vi "Wide Field Drift Correction.vi"(7 "Calling VI Ref":refnum<vi>) -> ()   [LabVIEW 2016]
uses:
  Hardware Configuration/Hardware Configuration Controls/Device Type.ctl
  Hardware Configuration/Hardware Configuration Controls/Device Function.ctl
  WFDC Controls/WFDC Notifier Element.ctl
  WFDC Controls/WFDC Actions.ctl
  <vilib>/vision/Image Controls.llb/IMAQ Image.ctl
  WFDC Controls/WFDC External Sync.ctl
  WFDC Controls/WFDC Cycle Pause.ctl
  WFDC Controls/WFDC Status.ctl
  WFDC Controls/WFDC Default XY Stage Settings.ctl
  <vilib>/Utility/miscctls.llb/LVPointTypeDef.ctl
  Device Library/Cameras/IDS/IDS Controls/IDS Actions.ctl
  Device Library/Cameras/IDS/IDS Controls/IDS Parameters.ctl
  Device Library/Cameras/IDS/IDS Controls/IDS Parameter List.ctl
  Device Library/Cameras/IDS/IDS Controls/IDS ROI.ctl
  Device Library/Cameras/IDS/IDS Controls/IDS IMAQ Key Info.ctl
  Device Library/Stages/Stages Controls/Stage Actions.ctl
  Tools/TIFF Image Read and Write/ImageJ TIF Type Defs/TIF Write Image Information.ctl
  Device Library/Cameras/Camera Controls/Camera IMAQ Key Info.ctl
panel:
  in  "Main Tab":T1(tab)
  out "Remote Start":bool
  out "Running":bool
  out "Z Drift (µm)":dbl=1.0 format="%.3g"
  out "Axis 2 Drift (Pixels)":dbl=1.0 format="%.3g"
  out "Axis 1 Drift (Pixels)":dbl=1.0 format="%.3g"
  out "Z Stage Position":dbl(graph)
  out "Z Drift Amount":dbl(graph)
  out "XY Drift Correction Active":bool
  out "Error":bool
  in  "Setup New":bool
  in  "Find Focus":bool
  in  "Z Step Correction Limit (µm)":dbl=0.2
  in  "Stage Defaults":bool
  in  "Invert Y Axis":bool
  in  "Invert X Axis":bool
  in  "Flip XY Axis":bool
  in  "Frame Accumulations":u16=20
  in  "Calibration Scan Range (µm)":dbl=1.0
  in  "Log Drift Data":bool
  in  "Save Drift Images":bool
  in  "Cycle Sync XY Correction":bool
  in  "Track XY Drift":bool
  in  "Correct XY Drift":bool
  in  "XY Drift Threshold (pixels)":dbl=0.2
  in  "XY Drift Step (µm)":dbl=0.1
  in  "Z Position Offset (µm)":dbl
  in  "Z Drift Threshold (µm)":dbl=0.02
  in  "Correct Z Drift":bool=TRUE
  in  "Abort Capture If Error":bool=TRUE
  in  "Cycle Sync Z Correction":bool
  out "XY Correction Step":i32=1
  out "Correction Step":u8=1
  in  "CC Range (pixels)":i32=25 min=1 max=200
  out "CC Fit":dbl[][](graph)
  out "CC Image":dbl[][](graph)
  in  "Abort Remote":bool
  in  "CC Threshold":dbl=0.2
  in  "Fit Roundess Threshold":dbl=1.75
  out "Axis 1":dbl=1.0 format="%.3g"
  out "Axis 2":dbl=1.0 format="%.3g"
  out "Z Drift":dbl=1.0 format="%.3g"
  out "Error Message":string
  out "XY Active":bool
  out "Z Active":bool
  out "Current Frame":u32=1
  in  "Capture":bool
  in  "Number of Frames":u32=1
  in  "Image Save Path":path
  in  "Exposure Time (ms)":dbl
  in  "Image Display":bool
  in  "Live Preview":bool
  in  "Quit":bool
  # "General Settings"
  # "XY Stage Settings"
  # "XY Drift Settings"
  # "Z Drift Settings"
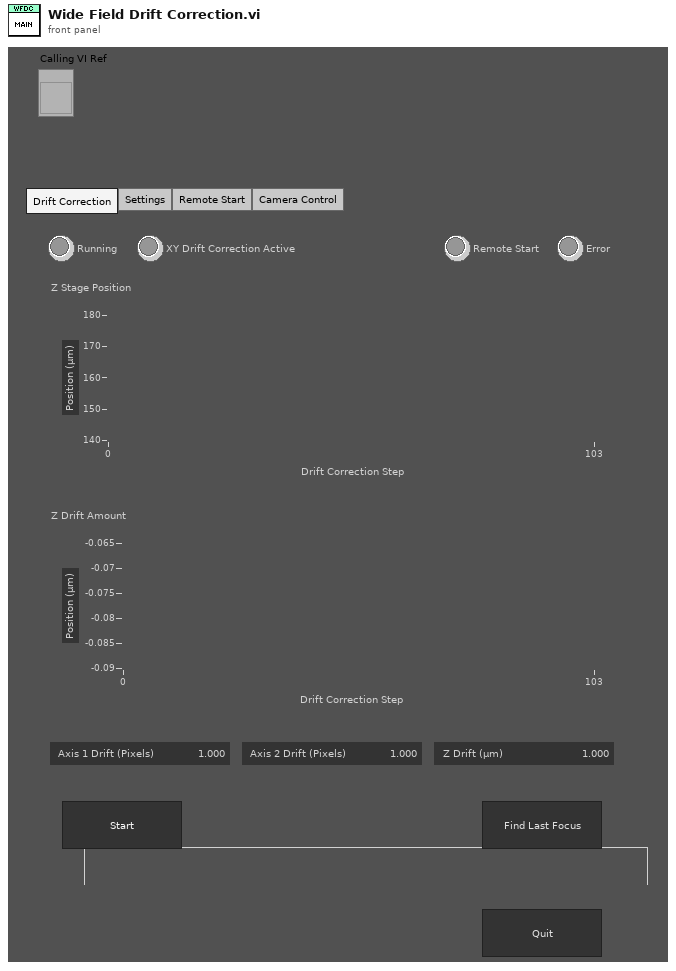
[diagram p1: front panel]
types:
  T1 = enum32{"Drift Correction", "Settings", "Remote Start", "Camera Control"}
  T2 = enum16{"Always On", "Always Off", "Off While Running"}
  T3 = typedef "LVPointTypeDef.ctl" = cluster{"Horizontal":i16, "Vertical":i16}
  T4 = typedef "IMAQ Image.ctl" = refnum<image>
  T5 = cluster{"Image Ref":T4, "Cycle Number":u16, "Camera Running?":bool, "Capture?":bool}
  T6 = typedef "WFDC Default XY Stage Settings.ctl" = cluster{"Flip XY":bool, "Invert X":bool, "Invert Y":bool}
  T7 = typedef "WFDC Cycle Pause.ctl" = enum16{"Pause Requested", "Paused", "Resume Requested", "Resumed"}
  T8 = typedef "WFDC Status.ctl" = enum16{"Idle", "Busy", "DC Active", "Error", "Canceled"}
  T9 = typedef "WFDC External Sync.ctl" = cluster{"Cycle Sync":T7, "Z Offset":dbl, "WFDC Status":T8}
  T10 = typedef "WFDC Actions.ctl" = enum16{"Error Check", "Remote Start", "Find Focus", "Pre Correct Z", "Pre Correct XY", "Setup New DC", "Setup Camera", "Get Ref Images", "Calc Calibration", "Setup Data Log", "Switch Tabs", "Get Drift / Correct Z", "Correct XY Drift", "Start Cycle", "Stop DC", "Abort Remote", "Exit Loop", "Set Error", "Generate Calibration", "Quit"}
  T11 = typedef "WFDC Notifier Element.ctl" = cluster{"WFDC Actions":T10, "Initial XYZ Positions":dbl[], "Ref Images":T4[], "Calibration (slope, inter)":dbl[], "Log Drift?":bool, "Save WF Images?":bool, "Drift Image File Ref":refnum<file>, "Drift Positions File Ref":refnum<file>, "Base Path":path, "Latest Scan Path":path, "Error":errorcluster}
  T12 = typedef "Device Function.ctl" = enum16{"Primary", "Secondary", "Overview", "Wide Field Drift Correction", "642 nm Excitation", "560 nm Excitation", "940 nm Excitation", "546 nm Excitation", "488 nm Excitation", "405 nm Excitation", "Objective Drift Correction", "4Pi Objective Lock", "Objective XY", "Objective Z", "Sample XY", "Sample Coarse Z", "Sample Z", "4Pi Lower", "4Pi Upper", "Mojo", "Adj Cavity", "Line Scanning", "Alert"}
  T13 = typedef "Device Type.ctl" = enum16{"AOTF", "Camera", "Deformable Mirror", "Laser", "Shutter", "Stage", "Waveform", "FPGA", "Email", "Filter Wheel"}
  T14 = typedef "LVRectTypeDef.ctl" = cluster{"Left":i16, "Top":i16, "Right":i16, "Bottom":i16}
  T15 = typedef "LVBoundsTypeDef.ctl" = cluster{"Width":u32, "Height":u32}
  T16 = enum8{"Enabled", "Disabled", "Disabled and Grayed Out"}
  T17 = typedef "IDS Actions.ctl" = enum16{"Error Check", "Initialize", "Preview", "Record", "Abort", "Record Settings", "Set Parameter", "Get Parameter", "Set ROI", "Get ROI", "Status", "Quit"}
  T18 = typedef "IDS Parameter List.ctl" = enum16{"Exposure Time (s)", "Binning"}
  T19 = typedef "IDS Parameters.ctl" = cluster{"Parameter":T18, "Value":dbl}
  T20 = typedef "IDS ROI.ctl" = cluster{"H Offset":i32, "V Offset":i32, "H Width":i32, "V Width":i32}
  T21 = typedef "IDS IMAQ Key Info.ctl" = cluster{"Frame":u32, "Sensor Height":i32, "Sensor Width":i32, "ROI Height":i32, "ROI Width":i32, "ROI Enable?":bool, "Bit per Pixel":u8}
  T22 = typedef "Stage Actions.ctl" = enum16{"Get Position", "MVR", "MOVE", "HALT", "ONTARGET", "ERROR", "REFERENCE", "INIT", "VELOCITY", "STATUS", "EXIT", "HOME", "ZEROPOS", "NANOPOS", "ANALOG", "QUIT"}
  T23 = enum16{"open", "replace", "create", "open or create", "replace or create", "replace or create with confirmation"}
  T24 = typedef "TIF Write Image Information.ctl" = cluster{"Image Width (Pixels)":u32, "Image Height (Pixels)":u32, "Pixel Width (µm)":dbl, "Pixel Height (µm)":dbl, "Bits Per Sample (e.g. 16)":u32, "No. of Frames":u32, "No. of Slices":u32, "Time Step (sec)":dbl, "Z Step (µm)":dbl}
  T25 = enum32{"Page Enabled", "Page Disabled", "Page Disabled & Grayed"}
  T26 = typedef "Camera IMAQ Key Info.ctl" = cluster{"Frame":u32, "Sensor Height":i32, "Sensor Width":i32, "ROI Height":i32, "ROI Width":i32, "ROI Enable?":bool, "Bit per Pixel":u8}
  T27 = enum16{"big-endian, network order", "native, host order", "little-endian"}
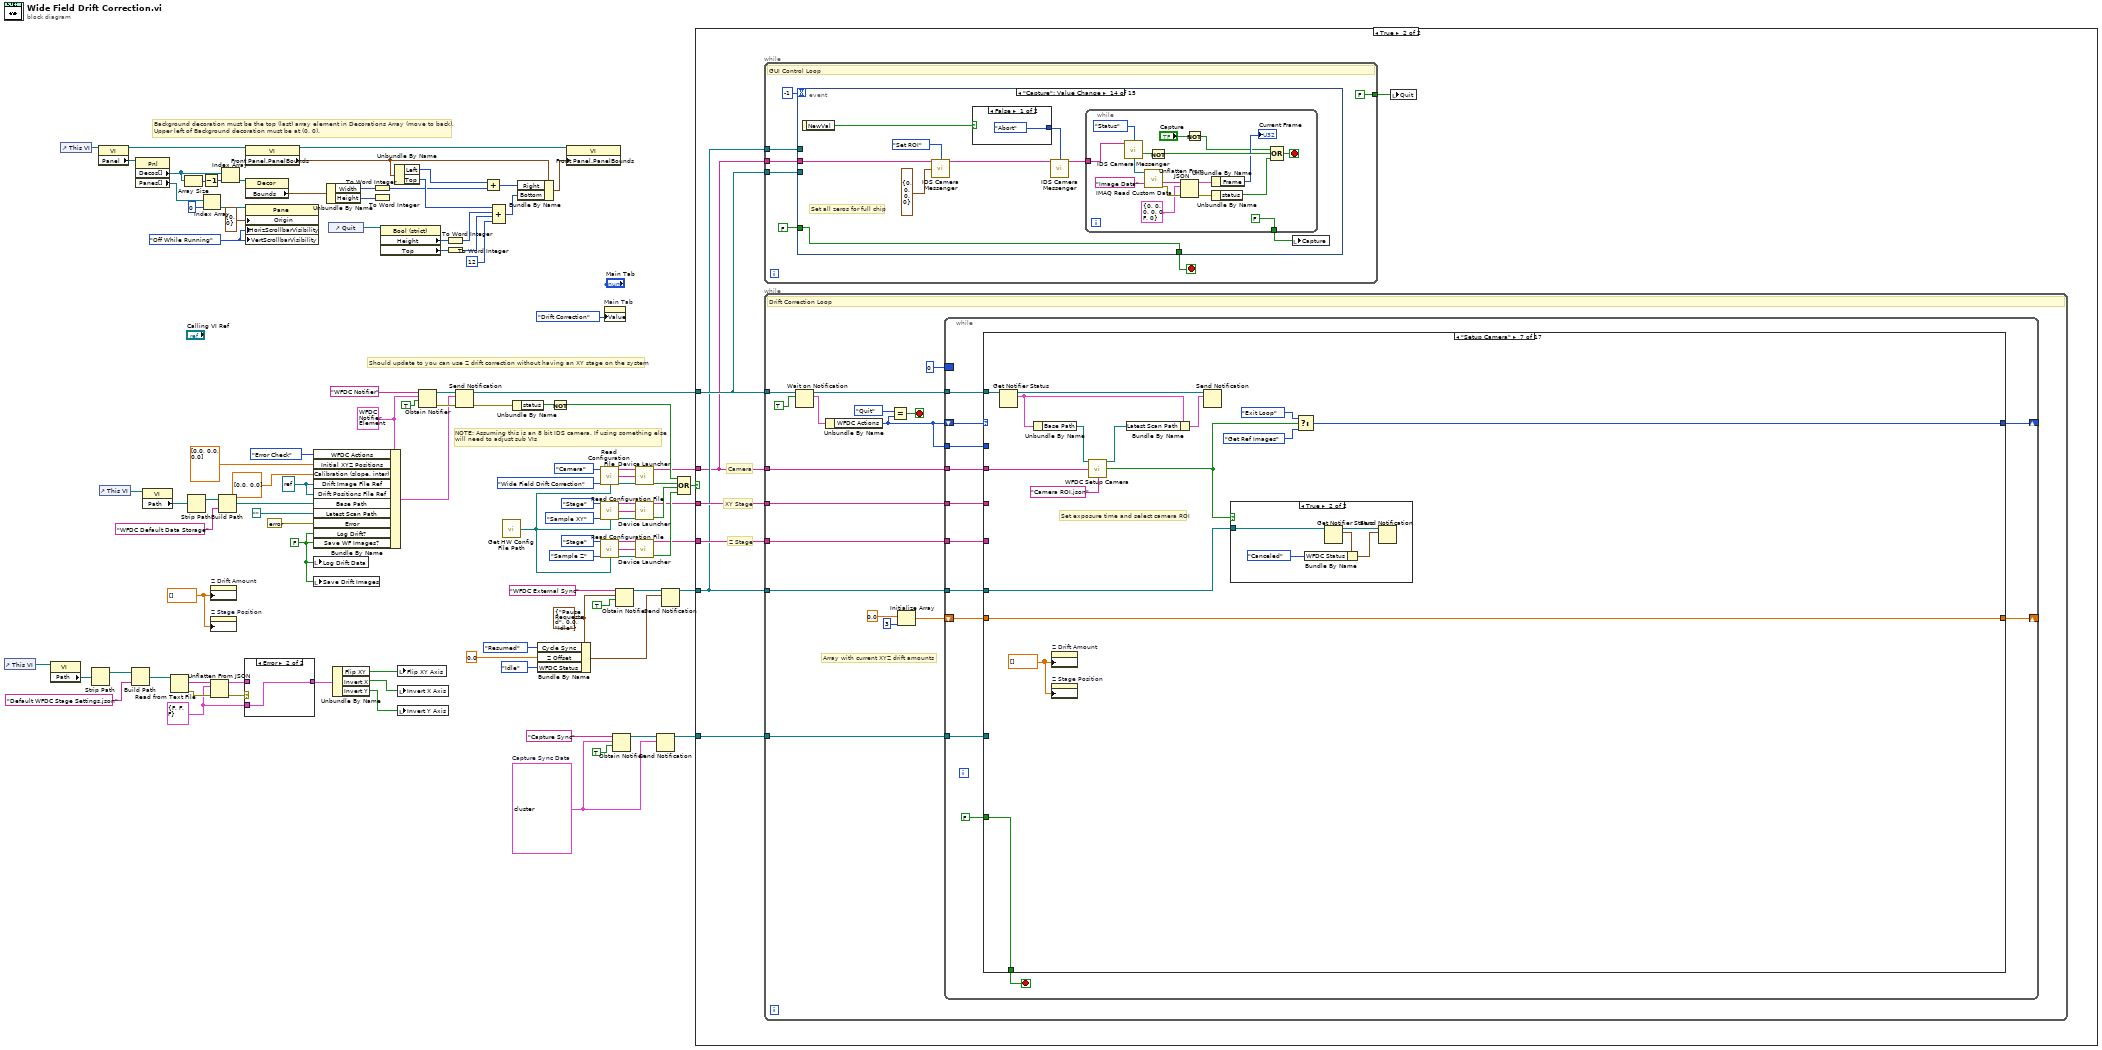
[diagram p0: block diagram]
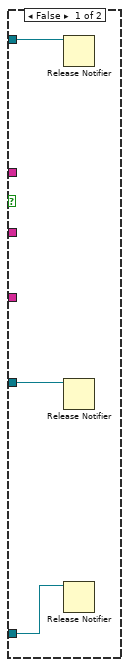
[diagram p3: hidden frame]
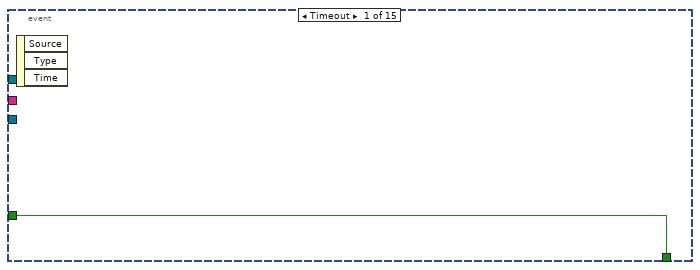
[diagram p4: hidden frame]
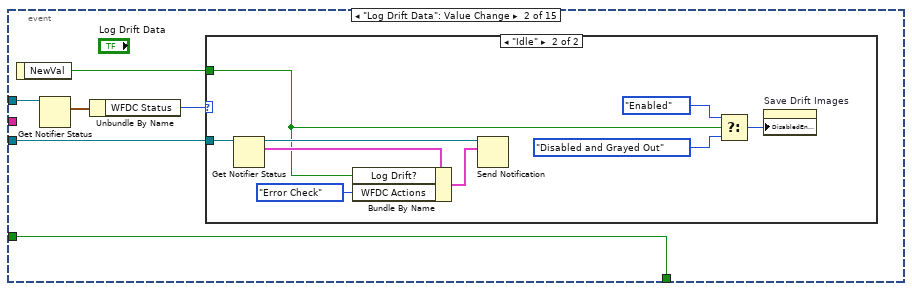
[diagram p5: hidden frame]
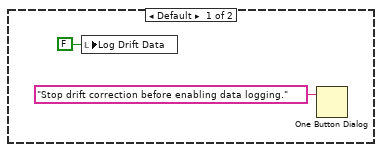
[diagram p6: hidden frame]
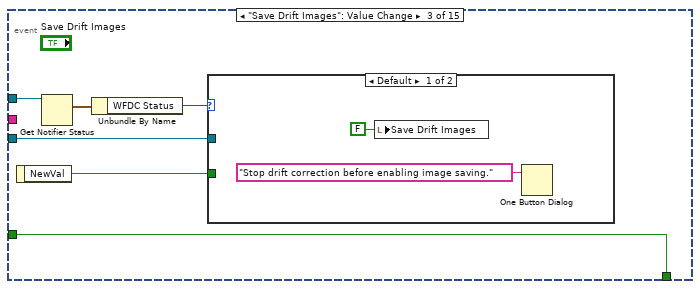
[diagram p7: hidden frame]
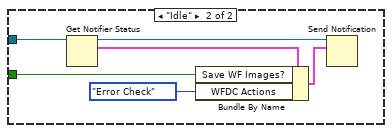
[diagram p8: hidden frame]
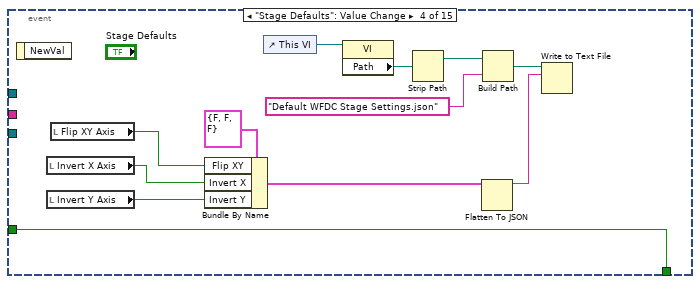
[diagram p9: hidden frame]
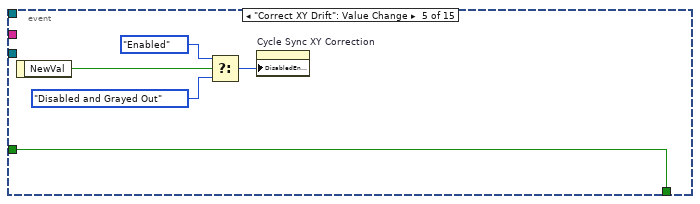
[diagram p10: hidden frame]
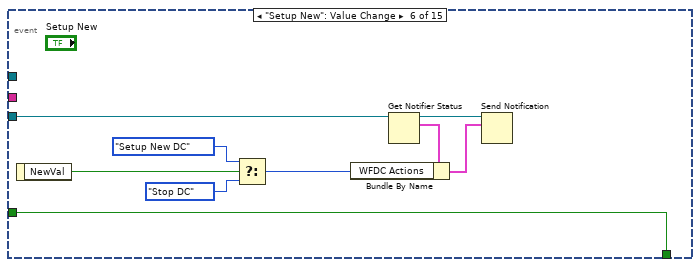
[diagram p11: hidden frame]
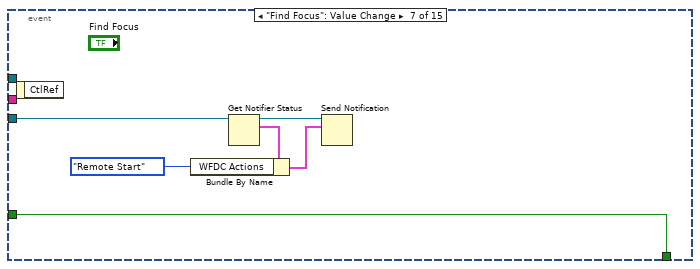
[diagram p12: hidden frame]
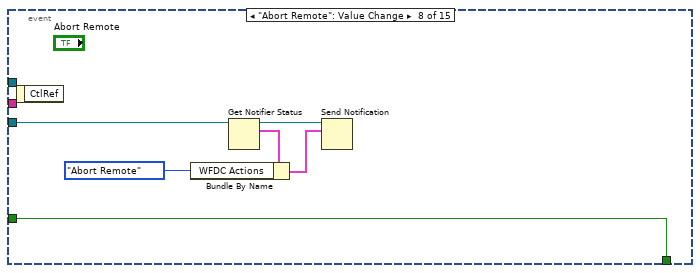
[diagram p13: hidden frame]
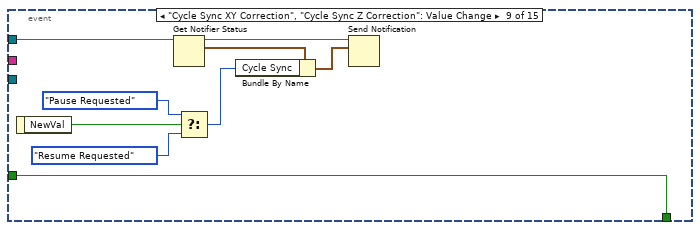
[diagram p14: hidden frame]
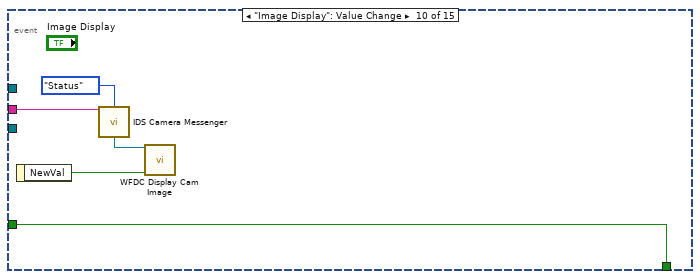
[diagram p15: hidden frame]
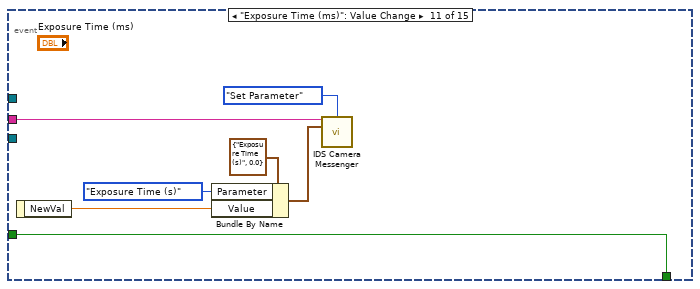
[diagram p16: hidden frame]
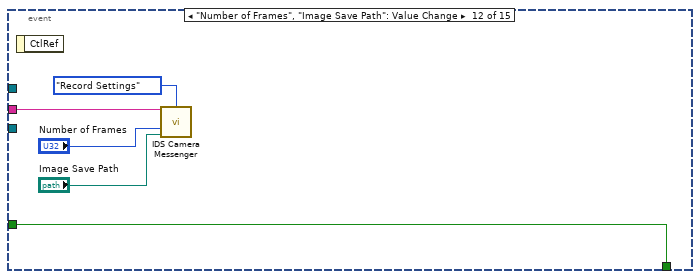
[diagram p17: hidden frame]
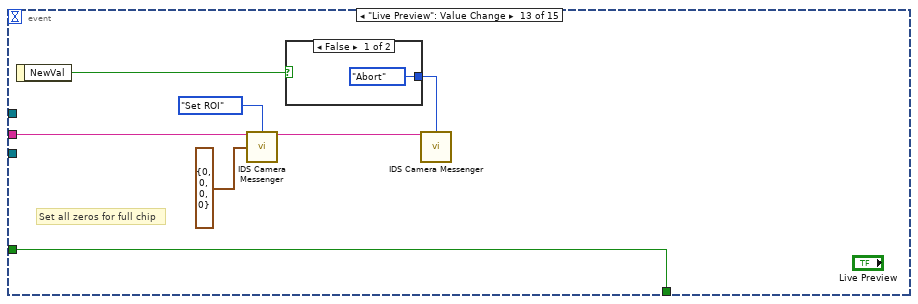
[diagram p18: hidden frame]
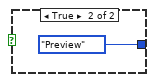
[diagram p19: hidden frame]
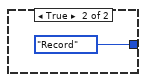
[diagram p20: hidden frame]
diagram:
  w13 = T2."Off While Running" ("Vertical Scrollbar Visibility")
  w46 = T5 {"Image Ref"=refnum, "Cycle Number"=0, "Camera Running?"=FALSE, "Capture?"=FALSE}  # Capture Sync Data
  w35 = T6 {"Flip XY"=FALSE, "Invert X"=FALSE, "Invert Y"=FALSE} ("Default WFDC Stage Settings")
  w56 = T9 {"Cycle Sync"=enum."Pause Requested", "Z Offset"=0.0, "WFDC Status"=enum."Idle"} ("WFDC External Sync")
  w64 = refnum<file> refnum ("Drift Image File Ref")
  w58 = FALSE ("Log Drift?")
  w68 = dbl[] []
  w70 = T11 {"WFDC Actions"=enum."Error Check", "Initial XYZ Positions"=[], "Ref Images"=[], "Calibration (slope, inter)"=[], "Log Drift?"=FALSE, "Save WF Images?"=FALSE, "Drift Image File Ref"=refnum, "Drift Positions File Ref"=refnum, "Base Path"=path "", "Latest Scan Path"=path "", "Error"={"status"=FALSE, "code"=0, "source"=""}} ("WFDC Notifier Element")
  # "Background decoration must be the top (last) array element in Decorations Array (move to back).\nUpper left of Background decoration must be at (0, 0)."
  # "Should update to you can use Z drift correction without having an XY stage on the system"
  # "NOTE: Assuming this is an 8 bit IDS camera. If using something else\nwill need to adjust sub VIs"
  n1 = control-ref of="This VI"() -> (w41:refnum<vi>)
  n2 = property class="VI"(reference=w41) -> ("Path"=w42:path)  [unwired: 1 in, 2 out]
  n3 = control-ref of="This VI"() -> (w5:refnum<vi>)
  n4 = Strip Path(path=w42) -> (stripped path=w43:path)  [unwired: 1 out]
  n5 = property class="VI"(reference=w5) -> (reference out=w14:refnum<vi>, "Panel"=w6:refnum<vi>)  [unwired: 1 in, 1 out]
  n6 = control-ref of="This VI"() -> (w104:refnum<vi>)
  n7 = Build Path(base path=w43, name or relative path="Default WFDC Stage Settings.json") -> (appended path=w40:path)
  n8 = property class="Pnl"(reference=w6) -> ("Decos[]"=w4:refnum<vi>[], "Panes[]"=w10:refnum<vi>[])  [unwired: 1 in, 2 out]
  n9 = property class="VI"(reference=w104) -> ("Path"=w103:path)  [unwired: 1 in, 2 out]
  n10 = Read from Text File(file (use dialog)=w40) -> (text=w39:string, error out=w38:errorcluster)  [unwired: 3 in, 2 out]
  n11 = Array Size(array=w4) -> (size(s)=w2:i32)
  n12 = Strip Path(path=w103) -> (stripped path=w102:path)  [unwired: 1 out]
  n13 = Decrement(x=w2) -> (x-1=w3:i32)
  n14 = Index Array(array=w10, index=0) -> (element=w9:refnum<vi>)
  n15 = property on="Z Drift Amount" class="WFChart (strict)"("History Data"=w68) -> ()  [unwired: 2 in, 2 out]
  n16 = property on="Z Stage Position" class="WFChart (strict)"("History Data"=w68) -> ()  [unwired: 2 in, 2 out]
  n17 = Unflatten From JSON(JSON string=w39, type and defaults=w35, error in (no error)=w38) -> (value=w36:T6, error out=w37:errorcluster)  [unwired: 4 in]
  n18 = Build Path(base path=w102, name or relative path="WFDC Default Data Storage") -> (appended path=w61:path)
  n19 = Index Array(array=w4, index=w3) -> (element=w12:refnum<vi>)
  n20 = case shown="Error" w37 {
    tunnel: w36 -> [w105 _]
    tunnel: [w105 w106] -> w34
    tunnel: w35 -> [_ w106]
    frame No Error {
    }
    frame Error {
    }
  }
  n21 = property class="VI"(reference=w14) -> (reference out=w16:refnum<vi>, "Front Panel.PanelBounds"=w17:T14)  [unwired: 1 in, 1 out]
  n22 = property class="Decor"(reference=w12) -> ("Bounds"=w15:T15)  [unwired: 1 in, 2 out]
  n23 = property class="Pane"(reference=w9, "Origin"=T3 {"Horizontal"=0, "Vertical"=0}, "HorizScrollbarVisibility"=w13, "VertScrollbarVisibility"=w13) -> ()  [unwired: 1 in, 2 out]
  n24 = Bundle By Name(cluster=w70, "WFDC Actions"=WFDC_Actions."Error Check", "Initial XYZ Positions"=dbl[] [0.0, 0.0, 0.0], "Calibration (slope, inter)"=dbl[] [0.0, 0.0], "Drift Image File Ref"=w64, "Drift Positions File Ref"=w64, "Base Path"=w61, "Latest Scan Path"=path "", "Error"=errorcluster {"status"=FALSE, "code"=0, "source"=""}, "Log Drift?"=w58, "Save WF Images?"=w58) -> (w69:T11)
  n25 = local write "Log Drift Data"(w58) -> ()
  n26 = local write "Save Drift Images"(w58) -> ()
  n27 = Unbundle By Name(w15) -> ("Width"=w20:u32, "Height"=w23:u32)
  n28 = control-ref of="Quit"() -> (w7:refnum<vi>)
  n29 = Unbundle By Name(w34) -> ("Flip XY"=w33:bool, "Invert X"=w32:bool, "Invert Y"=w31:bool)
  n30 = To Word Integer(number=w20) -> (16bit integer=w22:i16)
  n31 = To Word Integer(number=w23) -> ()  [unwired: 1 out]
  n32 = property class="Bool (strict)"(reference=w7) -> ("Height"=w25:u32, "Top"=w26:i32)  [unwired: 1 in, 2 out]
  n33 = Unbundle By Name(w17) -> ("Left"=w19:i16, "Top"=w30:i16)
  n34 = local write "Flip XY Axis"(w33) -> ()
  n35 = local write "Invert X Axis"(w32) -> ()
  n36 = local write "Invert Y Axis"(w31) -> ()
  n37 = Obtain Notifier(name (unnamed)="WFDC Notifier", notification data type=w70, create if not found? (T)=TRUE) -> (notifier out=w84:refnum<notifier>, error out=w82:errorcluster)  [unwired: 1 in, 1 out]
  n38 = To Word Integer(number=w25) -> (16bit integer=w28:i16)
  n39 = To Word Integer(number=w26) -> (16bit integer=w29:i16)
  n40 = Send Notification(notification=w69, notifier=w84, error in (no error)=w82) -> (notifier out=w83:refnum<notifier>, error out=w77:errorcluster)
  n41 = Add(x=w19, y=w22) -> (x+y=w21:i16)
  n42 = Compound Arithmetic op=ADD(w30, w28, w29, i16 12 ("y")) -> (w24:i16)
  n43 = call "Get HW Config File Path.vi"() -> ("File Path"=w66:path)  [unwired: 14 in, 1 out]
  n44 = Unbundle By Name(w77) -> ("status"=w76:bool)
  n45 = Bundle By Name(cluster=w17, "Right"=w21, "Bottom"=w24) -> (w18:T14)
  n46 = Bundle By Name(cluster=w56, "Cycle Sync"=WFDC_Cycle_Pause."Resumed", "Z Offset"=0.0, "WFDC Status"=WFDC_Status."Idle") -> (w50:T9)
  n47 = Not(x=w76) -> (.not. x?=w75:bool)
  n48 = property class="VI"(reference=w16, "Front Panel.PanelBounds"=w18) -> ()  [unwired: 1 in, 2 out]
  n49 = call "Read Configuration File.vi"("Device Type"=Device_Type."Camera", "Device Function"=Device_Function."Wide Field Drift Correction", "Config File Path"=w66) -> ("Unique Notifier Name"=w100:string, "Device Ports/IDs/Channels"=w99:string[], "Device Engine Path"=w98:path)  [unwired: 9 in, 1 out]
  n50 = call "Read Configuration File.vi"("Device Type"=Device_Type."Stage", "Device Function"=Device_Function."Sample XY", "Config File Path"=w66) -> ("Unique Notifier Name"=w91:string, "Device Ports/IDs/Channels"=w92:string[], "Device Engine Path"=w93:path)  [unwired: 9 in, 1 out]
  n51 = call "Read Configuration File.vi"("Device Type"=Device_Type."Stage", "Device Function"=Device_Function."Sample Z", "Config File Path"=w66) -> ("Unique Notifier Name"=w90:string, "Device Ports/IDs/Channels"=w89:string[], "Device Engine Path"=w88:path)  [unwired: 9 in, 1 out]
  n52 = property on="Main Tab" class="TabCtl (strict)"("Value"=T1."Drift Correction" ("Main Tab")) -> ()  [unwired: 2 in, 2 out]
  n53 = Obtain Notifier(name (unnamed)="Capture Sync", notification data type=w46, create if not found? (T)=TRUE) -> (notifier out=w47:refnum<notifier>)  [unwired: 1 in, 2 out]
  n54 = Obtain Notifier(name (unnamed)="WFDC External Sync", notification data type=w56, create if not found? (T)=TRUE) -> (notifier out=w52:refnum<notifier>)  [unwired: 1 in, 2 out]
  n55 = call "Device Launcher.vi"("Notifier Name"=w100, "Device Ports/IDs/Channels"=w99, "Device Engine Path"=w98) -> ("Notifier Name"=w73:string, "Running?"=w80:bool)  [unwired: 11 in]
  n56 = call "Device Launcher.vi"("Notifier Name"=w91, "Device Ports/IDs/Channels"=w92, "Device Engine Path"=w93) -> ("Notifier Name"=w72:string, "Running?"=w79:bool)  [unwired: 11 in]
  n57 = call "Device Launcher.vi"("Notifier Name"=w90, "Device Ports/IDs/Channels"=w89, "Device Engine Path"=w88) -> ("Notifier Name"=w71:string, "Running?"=w78:bool)  [unwired: 11 in]
  n58 = Send Notification(notification=w46, notifier=w47) -> (notifier out=w45:refnum<notifier>)  [unwired: 1 in, 1 out]
  n59 = Send Notification(notification=w50, notifier=w52) -> (notifier out=w51:refnum<notifier>)  [unwired: 1 in, 1 out]
  n60 = Compound Arithmetic op=OR(w75, w80, w79, w78) -> (w74:bool)
  n61 = case shown="True" w74 {
    tunnel: w83 -> [w109 w114]
    tunnel: w73 -> [_ w110]
    tunnel: w72 -> [_ w116]
    tunnel: w71 -> [_ w115]
    tunnel: w51 -> [w108 w112]
    tunnel: w45 -> [w107 w111]
    frame False {
      n62 = Release Notifier(notifier=w109) -> ()  [unwired: 2 in, 3 out]
      n63 = Release Notifier(notifier=w108) -> ()  [unwired: 2 in, 3 out]
      n64 = Release Notifier(notifier=w107) -> ()  [unwired: 2 in, 3 out]
    }
    frame True {
      # "Z Stage"
      # "XY Stage"
      # "Camera"
      n65 = while {
        tunnel: w114 -> [w120]
        tunnel: [FALSE] -> w113
        tunnel: w112 -> [w118]
        tunnel: w110 -> [w117]
        stop <- w123 stop-if-true
        # "GUI Control Loop"
        n66 = event shown="[13] \"Capture\": Value Change" {
          selector: _ -> [_ _ _ _ _ _ _ _ _ _ _ _ _ _ _]
          dyn-events: _ -> [_ _ _ _ _ _ _ _ _ _ _ _ _ _ _]
          timeout: -1 -> [_ _ _ _ _ _ _ _ _ _ _ _ _ _ _]
          tunnel: [w124 w130 w147 w167 w168 w181 w187 w193 w202 w205 w214 w219 w226 w230 w258] -> w123
          tunnel: FALSE -> [w124 w130 w147 w167 w168 w181 w187 w193 w202 w205 w214 w219 w226 w230 _]
          tunnel: w120 -> [_ w129 w146 _ _ w177 w182 w188 _ _ _ _ _ _ w264]
          tunnel: w118 -> [_ w127 w143 _ _ _ _ _ w200 _ _ _ _ _ w262]
          tunnel: w117 -> [_ _ _ _ _ _ _ _ _ w206 w209 w215 w221 w235 _]
          event Timeout {
            n67 = event-data() -> ()  [unwired: 1 in, 3 out]
          }
          event "Log Drift Data": Value Change {
            n68 = event-data() -> ("NewVal"=w128:bool)  [unwired: 1 in]
            n69 = Get Notifier Status(notifier=w127) -> (current notification=w126:T9)  [unwired: 1 in, 4 out]
            n70 = Unbundle By Name(w126) -> ("WFDC Status"=w125:T8)
            n71 = case shown="\"Idle\"" w125 {
              tunnel: w129 -> [_ w140]
              tunnel: w128 -> [_ w133]
              frame Default {
                n72 = local write "Log Drift Data"(FALSE ("Log Drift Data")) -> ()
                n73 = One Button Dialog(message="Stop drift correction before enabling data logging.") -> ()  [unwired: 1 in, 1 out]
              }
              frame "Idle" {
                n74 = Get Notifier Status(notifier=w140) -> (notifier out=w141:refnum<notifier>, current notification=w139:T11)  [unwired: 1 in, 3 out]
                n75 = Bundle By Name(cluster=w139, "Log Drift?"=w133, "WFDC Actions"=WFDC_Actions."Error Check") -> (w137:T11)
                n76 = Send Notification(notification=w137, notifier=w141) -> ()  [unwired: 1 in, 2 out]
                n77 = Select(t=T16."Enabled" ("Disabled"), s=w133, f=T16."Disabled and Grayed Out" ("Disabled")) -> (s? t:f=w134:T16)
                n78 = property on="Save Drift Images" class="Bool (strict)"("DisabledEnum"=w134) -> ()  [unwired: 2 in, 2 out]
              }
            }
          }
          event "Save Drift Images": Value Change {
            n79 = event-data() -> ("NewVal"=w145:bool)  [unwired: 1 in]
            n80 = Get Notifier Status(notifier=w143) -> (current notification=w144:T9)  [unwired: 1 in, 4 out]
            n81 = Unbundle By Name(w144) -> ("WFDC Status"=w142:T8)
            n82 = case shown="Default" w142 {
              tunnel: w146 -> [_ w154]
              tunnel: w145 -> [_ w152]
              frame Default {
                n83 = local write "Save Drift Images"(FALSE ("Save Drift Images")) -> ()
                n84 = One Button Dialog(message="Stop drift correction before enabling image saving.") -> ()  [unwired: 1 in, 1 out]
              }
              frame "Idle" {
                n85 = Get Notifier Status(notifier=w154) -> (notifier out=w155:refnum<notifier>, current notification=w153:T11)  [unwired: 1 in, 3 out]
                n86 = Bundle By Name(cluster=w153, "Save WF Images?"=w152, "WFDC Actions"=WFDC_Actions."Error Check") -> (w150:T11)
                n87 = Send Notification(notification=w150, notifier=w155) -> ()  [unwired: 1 in, 2 out]
              }
            }
          }
          event "Stage Defaults": Value Change {
            n88 = event-data() -> ()  [unwired: 1 in, 1 out]
            n89 = local read "Invert X Axis"() -> (w157:bool)
            n90 = local read "Invert Y Axis"() -> (w158:bool)
            n91 = local read "Flip XY Axis"() -> (w156:bool)
            n92 = Bundle By Name(cluster=T6 {"Flip XY"=FALSE, "Invert X"=FALSE, "Invert Y"=FALSE} ("Default WFDC Stage Settings"), "Flip XY"=w156, "Invert X"=w157, "Invert Y"=w158) -> (w159:T6)
            n93 = control-ref of="This VI"() -> (w166:refnum<vi>)
            n94 = property class="VI"(reference=w166) -> ("Path"=w165:path)  [unwired: 1 in, 2 out]
            n95 = Strip Path(path=w165) -> (stripped path=w164:path)  [unwired: 1 out]
            n96 = Flatten To JSON(anything=w159) -> (JSON string=w161:string)  [unwired: 2 in, 1 out]
            n97 = Build Path(base path=w164, name or relative path="Default WFDC Stage Settings.json") -> (appended path=w162:path)
            n98 = Write to Text File(file (use dialog)=w162, text=w161) -> ()  [unwired: 2 in, 3 out]
          }
          event "Correct XY Drift": Value Change {
            n99 = event-data() -> ("NewVal"=w172:bool)  [unwired: 1 in]
            n100 = Select(t=T16."Enabled" ("Disabled"), s=w172, f=T16."Disabled and Grayed Out") -> (s? t:f=w170:T16)
            n101 = property on="Cycle Sync XY Correction" class="Bool (strict)"("DisabledEnum"=w170) -> ()  [unwired: 2 in, 2 out]
          }
          event "Setup New": Value Change {
            n102 = event-data() -> ("NewVal"=w176:bool)  [unwired: 1 in]
            n103 = Select(t=WFDC_Actions."Setup New DC" ("WFDC Actions"), s=w176, f=WFDC_Actions."Stop DC" ("WFDC Actions")) -> (s? t:f=w174:T10)
            n104 = Get Notifier Status(notifier=w177) -> (notifier out=w179:refnum<notifier>, current notification=w180:T11)  [unwired: 1 in, 3 out]
            n105 = Bundle By Name(cluster=w180, "WFDC Actions"=w174) -> (w178:T11)
            n106 = Send Notification(notification=w178, notifier=w179) -> ()  [unwired: 1 in, 2 out]
          }
          event "Find Focus": Value Change {
            n107 = event-data() -> ()  [unwired: 1 in, 1 out]
            n108 = Get Notifier Status(notifier=w182) -> (notifier out=w185:refnum<notifier>, current notification=w186:T11)  [unwired: 1 in, 3 out]
            n109 = Bundle By Name(cluster=w186, "WFDC Actions"=WFDC_Actions."Remote Start") -> (w184:T11)
            n110 = Send Notification(notification=w184, notifier=w185) -> ()  [unwired: 1 in, 2 out]
          }
          event "Abort Remote": Value Change {
            n111 = event-data() -> ()  [unwired: 1 in, 1 out]
            n112 = Get Notifier Status(notifier=w188) -> (notifier out=w191:refnum<notifier>, current notification=w192:T11)  [unwired: 1 in, 3 out]
            n113 = Bundle By Name(cluster=w192, "WFDC Actions"=WFDC_Actions."Abort Remote") -> (w190:T11)
            n114 = Send Notification(notification=w190, notifier=w191) -> ()  [unwired: 1 in, 2 out]
          }
          event "Cycle Sync XY Correction", "Cycle Sync Z Correction": Value Change {
            n115 = event-data() -> ("NewVal"=w201:bool)  [unwired: 1 in]
            n116 = Get Notifier Status(notifier=w200) -> (notifier out=w195:refnum<notifier>, current notification=w199:T9)  [unwired: 1 in, 3 out]
            n117 = Select(t=WFDC_Cycle_Pause."Pause Requested" ("Cycle Sync"), s=w201, f=WFDC_Cycle_Pause."Resume Requested" ("Cycle Sync")) -> (s? t:f=w196:T7)
            n118 = Bundle By Name(cluster=w199, "Cycle Sync"=w196) -> (w194:T9)
            n119 = Send Notification(notification=w194, notifier=w195) -> ()  [unwired: 1 in, 2 out]
          }
          event "Image Display": Value Change {
            n120 = event-data() -> ("NewVal"=w203:bool)  [unwired: 1 in]
            n121 = call "IDS Camera Messenger.vi"("Notifier Name"=w206, "IDS Actions"=IDS_Actions."Status") -> ("Image Ref"=w204:T4)  [unwired: 8 in, 5 out]
            n122 = call "WFDC Display Cam Image.vi"("Image Ref"=w204, "Display?"=w203) -> ()  [unwired: 14 in]
          }
          event "Exposure Time (ms)": Value Change {
            n123 = event-data() -> ("NewVal"=w210:dbl)  [unwired: 1 in]
            n124 = Bundle By Name(cluster=T19 {"Parameter"=enum."Exposure Time (s)", "Value"=0.0} ("IDS Parameter"), "Parameter"=IDS_Parameter_List."Exposure Time (s)", "Value"=w210) -> (w208:T19)
            n125 = call "IDS Camera Messenger.vi"("Notifier Name"=w209, "IDS Actions"=IDS_Actions."Set Parameter", "IDS Parameter"=w208) -> ()  [unwired: 7 in, 6 out]
          }
          event "Number of Frames", "Image Save Path": Value Change {
            n126 = event-data() -> ()  [unwired: 1 in, 1 out]
            n127 = call "IDS Camera Messenger.vi"("Notifier Name"=w215, "IDS Actions"=IDS_Actions."Record Settings", "# of Frames"="Number of Frames", "File Save Path"="Image Save Path") -> ()  [unwired: 6 in, 6 out]
          }
          event "Live Preview": Value Change {
            # "Set all zeros for full chip"
            n128 = event-data() -> ("NewVal"=w225:bool)  [unwired: 1 in]
            n129 = call "IDS Camera Messenger.vi"("Notifier Name"=w221, "IDS Actions"=IDS_Actions."Set ROI", "ROI Setup"=T20 {"H Offset"=0, "V Offset"=0, "H Width"=0, "V Width"=0}) -> ("Notifier Name (Dup)"=w220:string)  [unwired: 7 in, 5 out]
            n130 = case shown="False" w225 {
              tunnel: [IDS_Actions."Abort" ("IDS Actions") IDS_Actions."Preview" ("IDS Actions")] -> w224
              frame False {
              }
              frame True {
              }
            }
            n131 = call "IDS Camera Messenger.vi"("Notifier Name"=w220, "IDS Actions"=w224) -> ()  [unwired: 8 in, 6 out]
          }
          event "Capture": Value Change {
            # "Set all zeros for full chip"
            n132 = event-data() -> ("NewVal"=w237:bool)  [unwired: 1 in]
            n133 = call "IDS Camera Messenger.vi"("Notifier Name"=w235, "IDS Actions"=IDS_Actions."Set ROI", "ROI Setup"=T20 {"H Offset"=0, "V Offset"=0, "H Width"=0, "V Width"=0}) -> ("Notifier Name (Dup)"=w234:string)  [unwired: 7 in, 5 out]
            n134 = case shown="False" w237 {
              tunnel: [IDS_Actions."Abort" ("IDS Actions") IDS_Actions."Record" ("IDS Actions")] -> w236
              frame False {
              }
              frame True {
              }
            }
            n135 = call "IDS Camera Messenger.vi"("Notifier Name"=w234, "IDS Actions"=w236) -> ("Notifier Name (Dup)"=w231:string)  [unwired: 8 in, 5 out]
            n136 = while {
              tunnel: w231 -> [w254]
              tunnel: [FALSE] -> w229
              stop <- w240 stop-if-true
              n137 = call "IDS Camera Messenger.vi"("Notifier Name"=w254, "IDS Actions"=IDS_Actions."Status") -> ("Running?"=w252:bool, "Image Ref"=w246:T4)  [unwired: 8 in, 4 out]
              n138 = call "IMAQ Read Custom Data"("Key"="Image Data", "Image"=w246) -> ("error out"=w251:errorcluster, "Custom Data Out"=w248:string)  [unwired: 7 in, 1 out]
              n139 = Not(x=w252) -> (.not. x?=w244:bool)
              n140 = Unflatten From JSON(JSON string=w248, type and defaults=T21 {"Frame"=0, "Sensor Height"=0, "Sensor Width"=0, "ROI Height"=0, "ROI Width"=0, "ROI Enable?"=FALSE, "Bit per Pixel"=0} ("IDS IMAQ Key Info"), error in (no error)=w251) -> (value=w250:T21, error out=w245:errorcluster)  [unwired: 4 in]
              n141 = Not(x="Capture") -> (.not. x?=w238:bool)
              n142 = Unbundle By Name(w250) -> ("Frame"=→"Current Frame":u32)
              n143 = Unbundle By Name(w245) -> ("status"=w243:bool)
              n144 = Compound Arithmetic op=OR(w238, w244, w243) -> (w240:bool)
            }
            n145 = local write "Capture"(w229) -> ()
          }
          event "Quit": Value Change {
            n146 = event-data() -> ()  [unwired: 1 in, 1 out]
            n147 = Get Notifier Status(notifier=w264) -> (notifier out=w263:refnum<notifier>, current notification=w266:T11)  [unwired: 1 in, 3 out]
            n148 = Bundle By Name(cluster=w266, "WFDC Actions"=WFDC_Actions."Stop DC", "Log Drift?"=FALSE) -> (w265:T11)
            n149 = Send Notification(notification=w265, notifier=w263) -> (notifier out=w261:refnum<notifier>)  [unwired: 1 in, 1 out]
            n150 = while {
              tunnel: w262 -> [w288]
              tunnel: w261 -> [w287]
              tunnel: [w287] -> w260
              tunnel: [w278] -> w259
              i -> [w281]
              stop <- w279 stop-if-true
              n151 = Get Notifier Status(notifier=w288) -> (current notification=w286:T9)  [unwired: 1 in, 4 out]
              n152 = Wait (ms)(milliseconds to wait=u32 1) -> ()  [unwired: 1 out]
              n153 = Greater?(x=w281, y=10000) -> (0:w278:bool)
              n154 = Unbundle By Name(w286) -> ("WFDC Status"=w285:T8)
              n155 = Equal?(x=WFDC_Status."Idle", y=w285) -> (x = y?=w282:bool)
              n156 = Or(x=w282, y=w278) -> (x .or. y?=w279:bool)
            }
            n157 = case shown="False" w259 {
              tunnel: w260 -> [w270 _]
              tunnel: [TRUE FALSE] -> w258
              frame False {
                n158 = flat-sequence {
                  tunnel: [w276] -> w271
                  tunnel: w270 -> [w276]
                  frame #0 {
                    n159 = Wait (ms)(milliseconds to wait=u32 20) -> ()  [unwired: 1 out]
                  }
                }
                n160 = Get Notifier Status(notifier=w271) -> (notifier out=w272:refnum<notifier>, current notification=w274:T11)  [unwired: 1 in, 3 out]
                n161 = Bundle By Name(cluster=w274, "WFDC Actions"=WFDC_Actions."Quit") -> (w269:T11)
                n162 = Send Notification(notification=w269, notifier=w272) -> ()  [unwired: 1 in, 2 out]
              }
              frame True {
              }
            }
          }
        }
      }
      n163 = while {
        tunnel: w114 -> [w304]
        tunnel: w110 -> [w296]
        tunnel: w116 -> [w299]
        tunnel: w115 -> [w298]
        tunnel: w112 -> [w291]
        tunnel: w111 -> [w290]
        stop <- w300 stop-if-true
        # "Array with current XYZ drift amounts"
        # "Drift Correction Loop"
        n164 = Wait on Notification(notifier=w304, ignore previous (F)=TRUE) -> (notifier out=w303:refnum<notifier>, notification=w302:T11)  [unwired: 2 in, 2 out]
        n165 = Unbundle By Name(w302) -> ("WFDC Actions"=w297:T10)
        n166 = Equal?(x=WFDC_Actions."Quit", y=w297) -> (x = y?=w300:bool)
        n167 = Initialize Array(0.0 ("element"), 3 ("dimension size")) -> (w294:dbl[])
        n168 = while {
          tunnel: w303 -> [w309]
          shift-right: [w313] -> _
          shift-left: w297 -> [w317]
          tunnel: w296 -> [w316]
          tunnel: w299 -> [w315]
          tunnel: w298 -> [w314]
          tunnel: w297 -> [w310]
          tunnel: w291 -> [w308]
          shift-right: [w306] -> _
          shift-left: w294 -> [w307]
          tunnel: w290 -> [w305]
          border: u8 0 -> [_]
          stop <- w311 stop-if-true
          n169 = case shown="\"Setup Camera\"" w317 {
            selector: w317 -> [_ _ _ _ _ _ _ _ _ _ _ _ _ _ w1062 _ _]
            tunnel: w316 -> [_ w356 w409 w472 w534 _ w683 w726 w762 w816 _ w912 _ _ w1077 _ _]
            tunnel: w315 -> [_ _ w396 w469 w541 _ _ w719 _ _ _ _ w971 _ _ _ _]
            tunnel: w314 -> [_ _ w408 w468 _ _ _ w716 _ _ _ w897 _ _ _ _ _]
            tunnel: [WFDC_Actions."Exit Loop" ("x") w350 w379 w461 w519 w663 w691 WFDC_Actions."Calc Calibration" ("x") w733 WFDC_Actions."Switch Tabs" ("x") WFDC_Actions."Get Drift / Correct Z" ("x") w855 w961 WFDC_Actions."Get Drift / Correct Z" ("x") WFDC_Actions."Exit Loop" ("x") WFDC_Actions."Exit Loop" ("x") WFDC_Actions."Quit" ("x")] -> w313
            tunnel: FALSE -> [w320 w372 w411 w476 w546 w664 w693 w727 w766 w817 w824 w916 w972 w1026 w1078 _ _]
            tunnel: [w320 w372 w411 w476 w546 w664 w693 w727 w766 w817 w824 w916 w972 w1026 w1078 TRUE TRUE] -> w311
            tunnel: w310 -> [_ _ _ _ _ w656 _ _ w737 _ _ _ _ _ _ _ _]
            tunnel: w309 -> [_ w371 w404 w475 w543 _ w687 w725 w765 w818 _ w915 _ _ w1074 _ w1094]
            tunnel: w308 -> [_ w341 w381 _ w536 w658 w679 _ w750 _ _ w886 w963 w1024 w1064 _ w1093]
            tunnel: w307 -> [w318 w342 w405 w470 w542 w662 w689 w706 w760 w809 w831 w908 w964 w1027 w1069 w1086 w1092]
            tunnel: [w318 w342 w405 w470 w542 w662 w689 w706 w760 w809 w831 w892 w964 w1027 w1069 w1086 w1092] -> w306
            tunnel: w305 -> [_ _ _ _ _ _ _ _ _ _ _ w883 _ w1023 _ _ w1089]
            frame "Error Check", Default {
            }
            frame "Remote Start" {
              n170 = Get Notifier Status(notifier=w371) -> (notifier out=w363:refnum<notifier>, current notification=w366:T11, error out=w351:errorcluster)  [unwired: 1 in, 2 out]
              n171 = Unbundle By Name(w366) -> ("Latest Scan Path"=w343:path)
              n172 = local write "Z Step Correction Limit (µm)"(10.0 ("Z Step Correction Limit (µm)")) -> ()
              n173 = Build Path(base path=w343, name or relative path="Scan Positions.xml") -> (appended path=w369:path)
              n174 = Build Path(base path=w343, name or relative path="Z Calibration.json") -> (appended path=w362:path)
              n175 = Build Path(base path=w343, name or relative path="Camera ROI.json") -> (appended path=w354:path)
              n176 = Build Path(base path=w343, name or relative path="Initial XYZ.json") -> (appended path=w340:path)
              n177 = call "WFDC Read Reference Images.vi"("Scan Positions File Path"=w369, "Error"=w351) -> ("Ref Images"=w365:T4[], "Error"=w358:errorcluster)  [unwired: 12 in]
              n178 = Read from Text File(file (use dialog)=w362, error in=w358) -> (refnum out=w337:refnum<file>, text=w361:string, error out=w333:errorcluster)  [unwired: 2 in, 1 out]
              n179 = Close File(refnum=w337, error in=w333) -> (error out=w330:errorcluster)  [unwired: 1 out]
              n180 = local write "Setup New"(TRUE ("Setup New")) -> ()
              n181 = Read from Text File(file (use dialog)=w354, error in=w330) -> (refnum out=w336:refnum<file>, text=w331:string, error out=w332:errorcluster)  [unwired: 2 in, 1 out]
              n182 = Close File(refnum=w336, error in=w332) -> (error out=w327:errorcluster)  [unwired: 1 out]
              n183 = Read from Text File(file (use dialog)=w340, error in=w327) -> (refnum out=w335:refnum<file>, text=w338:string, error out=w334:errorcluster)  [unwired: 2 in, 1 out]
              n184 = Close File(refnum=w335, error in=w334) -> (error out=w328:errorcluster)  [unwired: 1 out]
              n185 = local write "Error"(FALSE ("Error")) -> ()
              n186 = Unflatten From JSON(JSON string=w338, type and defaults=dbl[] [0.0, 0.0, 0.0], error in (no error)=w328) -> (value=w326:dbl[], error out=w329:errorcluster)  [unwired: 4 in]
              n187 = local write "Error Message"("") -> ()
              n188 = Unflatten From JSON(JSON string=w331, type and defaults=T20 {"H Offset"=0, "V Offset"=0, "H Width"=0, "V Width"=0} ("ROI Setup"), error in (no error)=w329) -> (value=w352:T20, error out=w353:errorcluster)  [unwired: 4 in]
              n189 = Unflatten From JSON(JSON string=w361, type and defaults=dbl[] [0.0, 0.0], error in (no error)=w353) -> (value=w359:dbl[], error out=w349:errorcluster)  [unwired: 4 in]
              n190 = call "IDS Camera Messenger.vi"("Notifier Name"=w356, "IDS Actions"=IDS_Actions."Set ROI", "ROI Setup"=w352) -> ()  [unwired: 7 in, 6 out]
              n191 = Bundle By Name(cluster=w366, "Ref Images"=w365, "Calibration (slope, inter)"=w359, "Error"=w349, "Initial XYZ Positions"=w326) -> (w364:T11)
              n192 = Send Notification(notification=w364, notifier=w363) -> ()  [unwired: 1 in, 2 out]
              n193 = case shown="No Error" w349 {
                tunnel: [WFDC_Actions."Find Focus" ("x") WFDC_Actions."Exit Loop" ("x")] -> w350
                tunnel: [WFDC_Status."Busy" ("WFDC Status") WFDC_Status."Error" ("WFDC Status")] -> w346
                frame No Error {
                }
                frame Error {
                }
              }
              n194 = Get Notifier Status(notifier=w341) -> (notifier out=w348:refnum<notifier>, current notification=w347:T9)  [unwired: 1 in, 3 out]
              n195 = Bundle By Name(cluster=w347, "WFDC Status"=w346) -> (w345:T9)
              n196 = Send Notification(notification=w345, notifier=w348) -> ()  [unwired: 1 in, 2 out]
              "Remote Start" <- TRUE ("Remote Start")
            }
            frame "Find Focus" {
              n197 = Get Notifier Status(notifier=w404) -> (current notification=w403:T11)  [unwired: 1 in, 4 out]
              n198 = Unbundle By Name(w403) -> ("Ref Images"=w402:T4[], "Initial XYZ Positions"=w395:dbl[])
              n199 = call "IDS Camera Messenger.vi"("Notifier Name"=w409, "IDS Actions"=IDS_Actions."Preview") -> ("Notifier Name (Dup)"=w385:string)  [unwired: 8 in, 5 out]
              n200 = Split 1D Array(array=w395, index=2) -> (first subarray=w393:dbl[], second subarray=w392:dbl[])
              n201 = disable-structure shown="Enabled" {
                disable-tunnel: w392 -> [w453 w454]
                disable-tunnel: [w451 w454] -> w389
                frame Disabled {
                  n202 = Subtract(x=w453, y=20.0) -> (x-y=w451:dbl[])
                }
                frame Enabled {
                }
              }
              n203 = Index Array(array=w402, index=1) -> (element=w386:T4)
              n204 = Greater Or Equal To 0?(x=w389) -> (x >= 0?=w391:bool[])
              n205 = And Array Elements(Boolean array=w391) -> (logical AND=w390:bool)
              n206 = call "Stages Messenger.vi"("Stage Notifier Name"=w396, "Actions"=Stage_Actions."MOVE", "Setpoint"=w393, "Axis"=bool[] [TRUE, TRUE], "Exit While Busy?"=FALSE) -> ()  [unwired: 7 in, 4 out]
              n207 = Select(t=w389, s=w390, f=dbl[] [0.0]) -> (s? t:f=w387:dbl[])
              n208 = call "Stages Messenger.vi"("Stage Notifier Name"=w408, "Actions"=Stage_Actions."MOVE", "Setpoint"=w387, "Axis"=bool[] [TRUE], "Exit While Busy?"=FALSE) -> ("Stage Notifier Name (Dup)"=w378:string)  [unwired: 7 in, 3 out]
              n209 = flat-sequence {
                tunnel: w378 -> [w456]
                tunnel: [w456] -> w377
                frame #0 {
                  n210 = Wait (ms)(milliseconds to wait=u32 350) -> ()  [unwired: 1 out]
                }
              }
              n211 = disable-structure shown="Enabled" {
                disable-tunnel: w386 -> [w421 _]
                disable-tunnel: w385 -> [w420 _]
                disable-tunnel: [w414 WFDC_Status."Busy" ("WFDC Status")] -> w380
                disable-tunnel: [w413 WFDC_Actions."Pre Correct Z" ("f")] -> w379
                disable-tunnel: w377 -> [w412 _]
                frame Disabled {
                  n212 = call "WFDC Scan Focus.vi"("Ref Image"=w421, "Camera Notifier"=w420, "Z Stage Notifier"=w412, "No. of Steps"=40, "Step Size (µm)"=1.0) -> ("Z Stage Notifier (Dup)"=w417:string, "Pos vs. Corr"=w416:dbl[][], "Canceled?"=w415:bool)  [unwired: 8 in]
                  n213 = case shown="False" w415 {
                    tunnel: [WFDC_Actions."Pre Correct Z" ("f") WFDC_Actions."Exit Loop" ("f")] -> w413
                    tunnel: w417 -> [w425 _]
                    tunnel: w416 -> [w424 _]
                    tunnel: [WFDC_Status."Busy" ("WFDC Status") WFDC_Status."Idle" ("WFDC Status")] -> w414
                    frame False {
                      n214 = Index Array(array=w424, index (col) #1=0 ("disabled index (col)"), index (col) #2=1 ("index (col)")) -> (element #1=w427:dbl[], element #2=w428:dbl[])  [unwired: 2 in]
                      n215 = disable-structure shown="Disabled" {
                        disable-tunnel: w428 -> [w434 w438]
                        disable-tunnel: w427 -> [w433 w439]
                        disable-tunnel: [w431 w435] -> w426
                        frame Enabled {
                          n216 = Array Max & Min(array=w434) -> (max index (indices)=w432:i32)  [unwired: 3 out]
                          n217 = Index Array(array=w433, index=w432) -> (element=w431:dbl)
                        }
                        frame Disabled {
                          n218 = call "1D Gaussian Fitting.vi"("X Values"=w439, "Y Values"=w438) -> ("Best Fit Parameters"=w437:dbl[])  [unwired: 11 in, 2 out]
                          n219 = Index Array(array=w437, index=1) -> (element=w435:dbl)
                        }
                      }
                      n220 = flat-sequence {
                        tunnel: w425 -> [w442]
                        tunnel: w426 -> [w441]
                        frame #0 {
                          n221 = Build Array(w441) -> (w440:dbl[])
                          n222 = call "Stages Messenger.vi"("Stage Notifier Name"=w442, "Actions"=Stage_Actions."MOVE", "Setpoint"=w440, "Axis"=bool[] [TRUE], "Exit While Busy?"=FALSE) -> ()  [unwired: 7 in, 4 out]
                        }
                        frame #1 {
                          n223 = Wait (ms)(milliseconds to wait=u32 350) -> ()  [unwired: 1 out]
                        }
                      }
                    }
                    frame True {
                    }
                  }
                }
                frame Enabled {
                }
              }
              n224 = Get Notifier Status(notifier=w381) -> (notifier out=w384:refnum<notifier>, current notification=w383:T9)  [unwired: 1 in, 3 out]
              n225 = Bundle By Name(cluster=w383, "WFDC Status"=w380) -> (w382:T9)
              n226 = Send Notification(notification=w382, notifier=w384) -> ()  [unwired: 1 in, 2 out]
            }
            frame "Pre Correct Z" {
              # "Limit the number of times to try to find the correct position."
              n227 = Get Notifier Status(notifier=w475) -> (current notification=w471:T11)  [unwired: 1 in, 4 out]
              n228 = Unbundle By Name(w471) -> ("Initial XYZ Positions"=w467:dbl[], "Calibration (slope, inter)"=w473:dbl[], "Ref Images"=w474:T4[])
              n229 = for {
                N: 3 -> [_]
                tunnel: w474 -> [w491]
                tunnel: w473 -> [w490]
                tunnel: w472 -> [w489]
                tunnel: w469 -> [w479]
                tunnel: w468 -> [w478]
                tunnel: w467 -> [w477]
                # "Initial Z Position"
                n230 = call "WFDC Get Current Image.vi"("IDS Camera Notifier Name"=w489, "Frames"=u16 20) -> ("Image - U16"=w486:u16[][], "Error"=w484:errorcluster)  [unwired: 11 in, 1 out]
                n231 = call "WFDC Get Current Drift.vi"("Ref Images"=w491, "Z Calibration (slope, inter)"=w490, "Half Shift"=11, "Current Image"=w486, "Error In"=w484, "Track XY Drift?"=FALSE) -> ("Z Position (µm)"=w485:dbl, "Error Out"=w480:errorcluster)  [unwired: 6 in, 2 out]
                n232 = Index Array(array=w477, index=2) -> (element=w482:dbl)
                n233 = case shown="No Error" w480 {
                  tunnel: w485 -> [w498 _]
                  tunnel: w482 -> [w497 _]
                  tunnel: w479 -> [_ w501]
                  tunnel: w478 -> [w493 w502]
                  tunnel: w477 -> [_ w510]
                  frame No Error {
                    n234 = Subtract(x=w497, y=w498) -> (x-y=w492:dbl)
                    "Z Drift" <- w492
                    n235 = Build Array(w492) -> (w496:dbl[])
                    n236 = call "Stages Messenger.vi"("Stage Notifier Name"=w493, "Actions"=Stage_Actions."MVR", "Setpoint"=w496, "Axis"=bool[] [TRUE]) -> ()  [unwired: 8 in, 4 out]
                  }
                  frame Error {
                    # "If there is a fitting error, set the stages to the initial positions."
                    n237 = Split 1D Array(array=w510, index=2) -> (first subarray=w504:dbl[], second subarray=w503:dbl[])
                    n238 = call "Stages Messenger.vi"("Stage Notifier Name"=w501, "Actions"=Stage_Actions."MOVE", "Setpoint"=w504, "Axis"=bool[] [TRUE, TRUE], "Exit While Busy?"=FALSE) -> ()  [unwired: 7 in, 4 out]
                    n239 = call "Stages Messenger.vi"("Stage Notifier Name"=w502, "Actions"=Stage_Actions."MOVE", "Setpoint"=w503, "Axis"=bool[] [TRUE], "Exit While Busy?"=FALSE) -> ()  [unwired: 7 in, 4 out]
                  }
                }
              }
              n240 = local write "XY Active"(FALSE ("XY Active")) -> ()
              n241 = feedback #1() -> (w457:u8)
              "Correction Step" <- w457
              n242 = Increment(x=w457) -> (x+1=w466:u8)
              n243 = feedback-in #1(w466) -> ()
              n244 = Greater?(x=w457, y=u8 50) -> (0:w464:bool)
              n245 = Select(t=WFDC_Actions."Set Error" ("x"), s=w464, f=WFDC_Actions."Pre Correct XY") -> (s? t:f=w461:T10)
              "Z Active" <- TRUE ("Z Active")
            }
            frame "Pre Correct XY" {
              n246 = Get Notifier Status(notifier=w543) -> (current notification=w544:T11)  [unwired: 1 in, 4 out]
              n247 = Unbundle By Name(w544) -> ("WFDC Actions"=w523:T10, "Log Drift?"=w525:bool, "Initial XYZ Positions"=w524:dbl[], "Ref Images"=w545:T4[])
              n248 = while {
                tunnel: w545 -> [w571]
                tunnel: w534 -> [w570]
                tunnel: w541 -> [w565]
                tunnel: w536 -> [w563]
                tunnel: [w563] -> w535
                tunnel: w524 -> [w562]
                tunnel: [w549] -> w516
                tunnel: [w548] -> w513
                i -> [w547]
                stop <- w558 stop-if-true
                n249 = call "WFDC Get Current Image.vi"("IDS Camera Notifier Name"=w570, "Frames"=u16 10) -> ("Image - U16"=w557:u16[][], "Error"=w569:errorcluster)  [unwired: 11 in, 1 out]
                n250 = local read "XY Drift Threshold (pixels)"() -> (w564:dbl)
                n251 = call "WFDC Get XY Drift.vi"("Ref Images"=w571, "Half Shift"="CC Range (pixels)", "Current Image"=w557, "CC Threshold"="CC Threshold", "Roundness Ratio"="Fit Roundess Threshold", "Error In"=w569) -> ("Axis 1 Drift (px)"=w554:dbl, "Axis 2 Drift (px)"=w553:dbl, "CC Image"=→"CC Image":dbl[][], "CC Fit"=→"CC Fit":dbl[][], "Error Out"=w567:errorcluster)  [unwired: 5 in]
                "Axis 2" <- w553
                "Axis 1" <- w554
                n252 = Build Array(w554, w553) -> (w566:dbl[])
                n253 = case shown="Error" w567 {
                  selector: w567 -> [_ w636]
                  tunnel: w565 -> [w585 w632]
                  tunnel: w566 -> [w584 _]
                  tunnel: [w573 w634] -> w560
                  tunnel: w564 -> [w581 _]
                  tunnel: w562 -> [_ w635]
                  tunnel: "CC Range (pixels)" -> [w580 _]
                  tunnel: [w574 w630] -> w549
                  frame No Error {
                    n254 = To Double Precision Float(number=w580) -> (double precision float=w579:dbl)
                    n255 = Multiply(x=w581, y=1.0) -> (x*y=w582:dbl)
                    n256 = Add(x=w582, y=w579) -> (x+y=w590:dbl)
                    n257 = Subtract(x=w579, y=w582) -> (x-y=w587:dbl)
                    n258 = for {
                      tunnel: w584 -> [w629] mode=indexing
                      tunnel: [w628] -> w592 mode=indexing
                      tunnel: w590 -> [w627]
                      tunnel: w587 -> [w626]
                      n259 = In Range and Coerce(upper limit=w627, x=w629, lower limit=w626) -> (In Range?=w628:bool)  [unwired: 1 out]
                    }
                    n260 = local read "Flip XY Axis"() -> (w596:bool)
                    n261 = local read "Invert X Axis"() -> (w597:bool)
                    n262 = local read "Invert Y Axis"() -> (w598:bool)
                    n263 = case shown="True" w596 {
                      tunnel: w584 -> [w607 w610]
                      tunnel: w592 -> [w606 w611]
                      tunnel: [w607 w609] -> w589
                      tunnel: [w606 w608] -> w588
                      frame False {
                      }
                      frame True {
                        n264 = Reverse 1D Array(array=w610) -> (reversed array=w609:dbl[])
                        n265 = Reverse 1D Array(array=w611) -> (reversed array=w608:bool[])
                      }
                    }
                    n266 = Build Array(w597, w598) -> (w593:bool[])
                    n267 = local read "XY Drift Step (µm)"() -> (w595:dbl)
                    n268 = for {
                      N: 2 -> [_]
                      tunnel: w588 -> [w624] mode=indexing
                      tunnel: w589 -> [w615] mode=indexing
                      tunnel: [w620] -> w578 mode=indexing
                      tunnel: [w623] -> w586 mode=indexing
                      tunnel: w590 -> [w622]
                      tunnel: w595 -> [w616]
                      tunnel: w593 -> [w617] mode=indexing
                      tunnel: w579 -> [w612]
                      n269 = Greater?(x=w615, y=w622) -> (0:w625:bool)
                      n270 = call "WFDC Dynamic Step.vi"("Setpoint"=w612, "Step Size"=w616, "Process Value"=w615, "Gain"=0.1) -> ("Output"=w614:dbl)  [unwired: 11 in]
                      n271 = Negate(x=w614) -> (-x=w621:dbl)
                      n272 = Not(x=w624) -> (.not. x?=w623:bool)
                      n273 = Select(t=w614, s=w625, f=w621) -> (s? t:f=w618:dbl)
                      n274 = Negate(x=w618) -> (-x=w619:dbl)
                      n275 = Select(t=w619, s=w617, f=w618) -> (s? t:f=w620:dbl)
                    }
                    n276 = And Array Elements(Boolean array=w592) -> (logical AND=w572:bool)
                    n277 = Not(x=w572) -> (.not. x?=w594:bool)
                    n278 = local write "XY Drift Correction Active"(w594) -> ()
                    n279 = Absolute Value(x=w578) -> (abs(x)=w577:dbl[])
                    n280 = Greater?(x=w577, y=3.0) -> (0:w575:bool[])
                    n281 = Or Array Elements(Boolean array=w575) -> (logical OR=w574:bool)
                    n282 = case shown="True" w574 {
                      tunnel: w586 -> [w603 _]
                      tunnel: w585 -> [w601 _]
                      tunnel: w578 -> [w600 _]
                      tunnel: [w599 TRUE] -> w573
                      tunnel: w572 -> [w599 _]
                      frame False {
                        n283 = call "Stages Messenger.vi"("Stage Notifier Name"=w601, "Actions"=Stage_Actions."MVR", "Setpoint"=w600, "Axis"=w603, "Exit While Busy?"=FALSE) -> ()  [unwired: 7 in, 4 out]
                      }
                      frame True {
                      }
                    }
                  }
                  frame Error {
                    # "-777 Initial guess outside image\n-776 CC intensity too low\n-775 Fit roundess\n-774 Fit result outside CC image"
                    n284 = Unbundle By Name(w636) -> ("code"=w633:i32, "source"=→"Error Message":string)
                    n285 = case shown="-777, -774" w633 {
                      tunnel: w632 -> [_ w644]
                      tunnel: w635 -> [_ w643]
                      tunnel: [w637 w638] -> w634
                      tunnel: [w637 w638] -> w630
                      frame Default {
                        w637 = TRUE
                      }
                      frame -777, -774 {
                        w638 = FALSE
                        n286 = Array Subset(array=w643, index=0, length=2) -> (w640:dbl[])
                        n287 = call "Stages Messenger.vi"("Stage Notifier Name"=w644, "Actions"=Stage_Actions."MOVE", "Setpoint"=w640, "Axis"=bool[] [TRUE, TRUE], "Exit While Busy?"=FALSE) -> ()  [unwired: 7 in, 4 out]
                      }
                    }
                  }
                }
                n288 = local read "Z Drift Threshold (µm)"() -> (w548:dbl)
                n289 = Greater Or Equal?(x=w547, y=15) -> (x >= y?=w559:bool)
                n290 = Or(x=w560, y=w559) -> (x .or. y?=w558:bool)
                "XY Correction Step" <- w547
              }
              n291 = Equal?(x=WFDC_Actions."Abort Remote", y=w523) -> (x = y?=w517:bool)
              n292 = Select(t=WFDC_Actions."Setup Data Log" ("x"), s=w525, f=WFDC_Actions."Switch Tabs" ("x")) -> (s? t:f=w538:T10)
              n293 = local write "Z Active"(FALSE ("Z Active")) -> ()
              n294 = local read "Cycle Sync XY Correction"() -> (w529:bool)
              n295 = local read "Cycle Sync Z Correction"() -> (w528:bool)
              n296 = Or(x=w517, y=w516) -> (x .or. y?=w515:bool)
              n297 = local read "Z Drift"() -> (w518:dbl)
              n298 = Or(x=w529, y=w528) -> (x .or. y?=w527:bool)
              n299 = Absolute Value(x=w518) -> (abs(x)=w533:dbl)
              n300 = Less Or Equal?(x=w533, y=w513) -> (x <= y?=w511:bool)
              n301 = Select(t=w538, s=w511, f=WFDC_Actions."Pre Correct Z") -> (s? t:f=w520:T10)
              n302 = Select(t=WFDC_Actions."Set Error", s=w515, f=w520) -> (s? t:f=w519:T10)
              n303 = Not(x=w511) -> (.not. x?=w532:bool)
              n304 = Select(t=WFDC_Cycle_Pause."Pause Requested" ("Cycle Sync"), s=w527, f=WFDC_Cycle_Pause."Resume Requested" ("Cycle Sync")) -> (s? t:f=w526:T7)
              n305 = case shown="True" w511 {
                tunnel: w535 -> [_ w649]
                tunnel: w526 -> [_ w648]
                frame False {
                }
                frame True {
                  w647 = FALSE ("Z Active")
                  n306 = local write "Z Active"(w647) -> ()
                  n307 = local write "XY Active"(w647) -> ()
                  n308 = Get Notifier Status(notifier=w649) -> (notifier out=w650:refnum<notifier>, current notification=w651:T9)  [unwired: 1 in, 3 out]
                  n309 = Bundle By Name(cluster=w651, "WFDC Status"=WFDC_Status."DC Active", "Cycle Sync"=w648) -> (w652:T9)
                  n310 = Send Notification(notification=w652, notifier=w650) -> ()  [unwired: 1 in, 2 out]
                }
              }
              n311 = local write "Running"(w511) -> ()
              n312 = local write "Remote Start"(w532) -> ()
              "XY Active" <- TRUE ("XY Active")
            }
            frame "Setup New DC", "Generate Calibration" {
              n313 = case shown="\"Generate Calibration\", Default" w656 {
                tunnel: [WFDC_Actions."Setup Camera" ("f") w668] -> w663
                frame "Generate Calibration", Default {
                }
                frame "Setup New DC" {
                  n314 = Two Button Dialog(message="Is the Z stage is near its center position?", 1:"No" ("F button name (\"Cancel\")"), 2:"Yes" ("T button name (\"OK\")")) -> (T button?=w671:bool)
                  n315 = case shown="False" w671 {
                    selector: w671 -> [w675 w677]
                    tunnel: "Center Z Stage and start again" ("message") -> [w676 _]
                    tunnel: [w675 w677] -> w666
                    frame False {
                      n316 = One Button Dialog(message=w676) -> ()  [unwired: 1 in, 1 out]
                    }
                    frame True {
                    }
                  }
                  n317 = Select(t=WFDC_Actions."Setup Camera" ("x"), s=w666, f=WFDC_Actions."Exit Loop") -> (s? t:f=w668:T10)
                }
              }
              n318 = Get Notifier Status(notifier=w658) -> (notifier out=w660:refnum<notifier>, current notification=w659:T9)  [unwired: 1 in, 3 out]
              n319 = Bundle By Name(cluster=w659, "WFDC Status"=WFDC_Status."Busy") -> (w661:T9)
              n320 = local write "Error"(FALSE ("Error")) -> ()
              n321 = Send Notification(notification=w661, notifier=w660) -> ()  [unwired: 1 in, 2 out]
              "Running" <- TRUE ("Running")
            }
            frame "Setup Camera" {
              w690 = dbl[] []
              # "Set exposure time and select camera ROI"
              n322 = Get Notifier Status(notifier=w687) -> (notifier out=w688:refnum<notifier>, current notification=w686:T11)  [unwired: 1 in, 3 out]
              n323 = Unbundle By Name(w686) -> ("Base Path"=w682:path)
              n324 = property on="Z Drift Amount" class="WFChart (strict)"("History Data"=w690) -> ()  [unwired: 2 in, 2 out]
              n325 = property on="Z Stage Position" class="WFChart (strict)"("History Data"=w690) -> ()  [unwired: 2 in, 2 out]
              n326 = call "WFDC Setup Camera.vi"("Base Data Path"=w682, "Camera Notifier Name"=w683, "ROI File Name"="Camera ROI.json" ("name or relative path")) -> ("Current Save Path"=w684:path, "Canceled?"=w678:bool)  [unwired: 11 in]
              n327 = Bundle By Name(cluster=w686, "Latest Scan Path"=w684) -> (w685:T11)
              n328 = Send Notification(notification=w685, notifier=w688) -> ()  [unwired: 1 in, 2 out]
              n329 = case shown="True" w678 {
                tunnel: w679 -> [_ w694]
                frame False {
                }
                frame True {
                  n330 = Get Notifier Status(notifier=w694) -> (notifier out=w697:refnum<notifier>, current notification=w696:T9)  [unwired: 1 in, 3 out]
                  n331 = Bundle By Name(cluster=w696, "WFDC Status"=WFDC_Status."Canceled") -> (w698:T9)
                  n332 = Send Notification(notification=w698, notifier=w697) -> ()  [unwired: 1 in, 2 out]
                }
              }
              n333 = Select(t=WFDC_Actions."Exit Loop", s=w678, f=WFDC_Actions."Get Ref Images" ("y")) -> (s? t:f=w691:T10)
            }
            frame "Get Ref Images" {
              n334 = call "Stages Messenger.vi"("Stage Notifier Name"=w719, "Actions"=Stage_Actions."Get Position") -> ("Positions"=w711:dbl[])  [unwired: 10 in, 3 out]
              n335 = call "Stages Messenger.vi"("Stage Notifier Name"=w716, "Actions"=Stage_Actions."Get Position") -> ("Stage Notifier Name (Dup)"=w715:string, "Positions"=w714:dbl[])  [unwired: 10 in, 2 out]
              n336 = Index Array(array=w711, index #1=0 ("index"), index #2=1 ("index")) -> (element #1=w709:dbl, element #2=w708:dbl)
              n337 = Index Array(array=w714, index=0) -> (element=w707:dbl)
              n338 = Get Notifier Status(notifier=w725) -> (notifier out=w723:refnum<notifier>, current notification=w722:T11)  [unwired: 1 in, 3 out]
              n339 = Unbundle By Name(w722) -> ("Latest Scan Path"=w702:path)
              n340 = Build Array(w709, w708, w707) -> (w703:dbl[])
              n341 = call "WFDC Get Reference Images.vi"("IDS Camera Notifier"=w726, "Data Save Path"=w702, "Z Stage Notifier"=w715, "Scan Range"="Calibration Scan Range (µm)", "Frame per Step"=u32 20, "Scan Positions File Name"="Scan Positions.xml" ("name or relative path")) -> ()  [unwired: 10 in]
              n342 = Build Path(base path=w702, name or relative path="Initial XYZ.json") -> (appended path=w700:path)
              n343 = Flatten To JSON(anything=w703) -> (JSON string=w699:string)  [unwired: 2 in, 1 out]
              n344 = Bundle By Name(cluster=w722, "Initial XYZ Positions"=w703) -> (w721:T11)
              n345 = Write to Text File(file (use dialog)=w700, text=w699) -> ()  [unwired: 2 in, 3 out]
              n346 = Send Notification(notification=w721, notifier=w723) -> ()  [unwired: 1 in, 2 out]
            }
            frame "Calc Calibration" {
              n347 = Get Notifier Status(notifier=w765) -> (notifier out=w732:refnum<notifier>, current notification=w764:T11)  [unwired: 1 in, 3 out]
              n348 = flat-sequence {
                tunnel: w764 -> [w781]
                tunnel: [w779] -> w763
                tunnel: w762 -> [w776]
                tunnel: [w776] -> w761
                tunnel: [w774] -> w736
                tunnel: [w773] -> w751
                tunnel: w750 -> [w773]
                tunnel: [w771] -> w745
                tunnel: [w770] -> w746
                tunnel: w739 -> [w769]
                frame #0 {
                  n349 = Unbundle By Name(w781) -> ("Latest Scan Path"=w771:path, "Log Drift?"=w774:bool)
                  n350 = call "WFDC Compute Z Calibration.vi"("Scan Positions File Name"="Scan Positions.xml" ("name or relative path"), "User Close?"=w769, "Half Shift"=7, "Data Path"=w771) -> ("Fit Slope"=w780:dbl, "Fit Intercept"=w778:dbl, "Ref Images"=w775:T4[], "Error"=w777:errorcluster)  [unwired: 8 in]
                  n351 = Build Array(w780, w778) -> (w770:dbl[])
                  n352 = Bundle By Name(cluster=w781, "Calibration (slope, inter)"=w770, "Error"=w777, "Ref Images"=w775) -> (w779:T11)
                }
              }
              n353 = Equal?(x=WFDC_Actions."Generate Calibration", y=w737) -> (x = y?=w728:bool)
              n354 = Equal?(x=WFDC_Actions."Setup New DC", y=w737) -> (x = y?=w739:bool)
              n355 = Send Notification(notification=w763, notifier=w732) -> ()  [unwired: 1 in, 2 out]
              n356 = Flatten To JSON(anything=w746) -> (JSON string=w742:string)  [unwired: 2 in, 1 out]
              n357 = Build Path(base path=w745, name or relative path="Z Calibration.json") -> (appended path=w743:path)
              n358 = Write to Text File(file (use dialog)=w743, text=w742) -> (refnum out=w741:refnum<file>)  [unwired: 2 in, 2 out]
              n359 = Close File(refnum=w741) -> ()  [unwired: 1 in, 2 out]
              n360 = Select(t=WFDC_Actions."Setup Data Log" ("x"), s=w736, f=WFDC_Actions."Switch Tabs" ("x")) -> (s? t:f=w735:T10)
              n361 = local read "Cycle Sync XY Correction"() -> (w749:bool)
              n362 = local read "Cycle Sync Z Correction"() -> (w748:bool)
              n363 = case shown="True" w728 {
                tunnel: w761 -> [w768 _]
                frame False {
                  # "Start Camera"
                  n364 = call "IDS Camera Messenger.vi"("Notifier Name"=w768, "IDS Actions"=IDS_Actions."Preview") -> ()  [unwired: 8 in, 6 out]
                }
                frame True {
                }
              }
              n365 = Select(t=WFDC_Actions."Exit Loop", s=w728, f=w735) -> (s? t:f=w733:T10)
              n366 = Or(x=w749, y=w748) -> (x .or. y?=w747:bool)
              n367 = Select(t=WFDC_Cycle_Pause."Pause Requested" ("Cycle Sync"), s=w747, f=WFDC_Cycle_Pause."Resumed" ("Cycle Sync")) -> (s? t:f=w755:T7)
              n368 = Select(t=WFDC_Status."Idle" ("WFDC Status"), s=w728, f=WFDC_Status."DC Active" ("WFDC Status")) -> (s? t:f=w730:T8)
              n369 = Get Notifier Status(notifier=w751) -> (notifier out=w759:refnum<notifier>, current notification=w758:T9)  [unwired: 1 in, 3 out]
              n370 = Bundle By Name(cluster=w758, "Cycle Sync"=w755, "WFDC Status"=w730) -> (w757:T9)
              n371 = Send Notification(notification=w757, notifier=w759) -> ()  [unwired: 1 in, 2 out]
            }
            frame "Setup Data Log" {
              w804 = 1.0 ("Pixel Width (µm)")
              n372 = Get Notifier Status(notifier=w818) -> (notifier out=w814:refnum<notifier>, current notification=w815:T11)  [unwired: 1 in, 3 out]
              n373 = Unbundle By Name(w815) -> ("Latest Scan Path"=w783:path, "Save WF Images?"=w810:bool)
              n374 = call "IDS Camera Messenger.vi"("Notifier Name"=w816, "IDS Actions"=IDS_Actions."Status") -> ("Image Ref"=w799:T4)  [unwired: 8 in, 5 out]
              n375 = Build Path(base path=w783, name or relative path="Drift Images.tif") -> (appended path=w806:path)
              n376 = call "IMAQ Read Custom Data"("Key"="Image Data", "Image"=w799) -> ("error out"=w798:errorcluster, "Custom Data Out"=w795:string)  [unwired: 7 in, 1 out]
              n377 = Build Path(base path=w783, name or relative path="Drift Positions.txt") -> (appended path=w787:path)
              n378 = Unflatten From JSON(JSON string=w795, type and defaults=T21 {"Frame"=0, "Sensor Height"=0, "Sensor Width"=0, "ROI Height"=0, "ROI Width"=0, "ROI Enable?"=FALSE, "Bit per Pixel"=0} ("IDS IMAQ Key Info"), error in (no error)=w798) -> (value=w793:T21)  [unwired: 4 in, 1 out]
              n379 = Unbundle By Name(w793) -> ("ROI Width"=w792:i32, "ROI Height"=w791:i32)  [unwired: 1 out]
              n380 = Open/Create/Replace File(file path (use dialog)=w787, operation (0:open)=T23."create", access (0:read/write)=enum16{"read/write", "read-only", "write-only"}."write-only") -> (refnum out=w811:refnum<file>)  [unwired: 3 in, 2 out]
              n381 = To Unsigned Long Integer(number=w792) -> (unsigned 32bit integer=w790:u32)
              n382 = To Unsigned Long Integer(number=w791) -> (unsigned 32bit integer=w789:u32)
              n383 = Bundle By Name(cluster=T24 {"Image Width (Pixels)"=0, "Image Height (Pixels)"=0, "Pixel Width (µm)"=0.0, "Pixel Height (µm)"=0.0, "Bits Per Sample (e.g. 16)"=0, "No. of Frames"=0, "No. of Slices"=0, "Time Step (sec)"=0.0, "Z Step (µm)"=0.0} ("Image Info"), "Image Width (Pixels)"=w790, "Image Height (Pixels)"=w789, "Pixel Width (µm)"=w804, "Pixel Height (µm)"=w804, "Bits Per Sample (e.g. 16)"=u32 16, "No. of Frames"=u32 1000000000, "No. of Slices"=u32 0, "Time Step (sec)"=0.0, "Z Step (µm)"=0.0) -> (w788:T24)
              n384 = case shown="True" w810 {
                tunnel: w806 -> [_ w823]
                tunnel: w788 -> [_ w822]
                tunnel: [refnum<file> refnum ("File Ref") w821] -> w812
                frame False {
                }
                frame True {
                  n385 = call "Write TIFF Header.vi"("File Path"=w823, "Image Info"=w822) -> ("File Ref"=w821:refnum<file>)  [unwired: 11 in, 2 out]
                }
              }
              n386 = Bundle By Name(cluster=w815, "Drift Image File Ref"=w812, "Drift Positions File Ref"=w811) -> (w813:T11)
              n387 = Send Notification(notification=w813, notifier=w814) -> ()  [unwired: 1 in, 2 out]
            }
            frame "Switch Tabs" {
              n388 = property on="Main Tab" class="TabCtl (strict)"("Value"=T1."Drift Correction" ("Main Tab")) -> ("Pages"=w828:refnum<vi>[])  [unwired: 2 in, 2 out]
              n389 = Index Array(array=w828, index=3) -> (element=w826:refnum<vi>)
              n390 = property class="Page"(reference=w826, "PageEnb"=T25."Page Disabled & Grayed" ("Page Enabled State")) -> ()  [unwired: 1 in, 2 out]
            }
            frame "Get Drift / Correct Z" {
              w887 = WFDC_Actions."Stop DC" ("x")
              # "This has turned into a giant shit show, again. Need to clean up!"
              # "Initial Z Position"
              n391 = Get Notifier Status(notifier=w915) -> (current notification=w891:T11)  [unwired: 1 in, 4 out]
              n392 = Get Notifier Status(notifier=w886) -> (current notification=w885:T9)  [unwired: 1 in, 4 out]
              n393 = Unbundle By Name(w885) -> ("Z Offset"=w884:dbl, "Cycle Sync"=w849:T7)
              n394 = Unbundle By Name(w891) -> ("WFDC Actions"=w888:T10, "Initial XYZ Positions"=w898:dbl[], "Calibration (slope, inter)"=w913:dbl[], "Ref Images"=w914:T4[])
              n395 = Equal?(x=w849, y=WFDC_Cycle_Pause."Paused") -> (x = y?=w844:bool)
              n396 = call "WFDC Get Current Image.vi"("IDS Camera Notifier Name"=w912, "Frames"="Frame Accumulations") -> ("Image - U16"=w870:u16[][], "Error"=w868:errorcluster)  [unwired: 11 in, 1 out]
              n397 = Equal?(x=w887, y=w888) -> (x = y?=w857:bool)
              n398 = Get Notifier Status(notifier=w883) -> (current notification=w882:T5, error out=w858:errorcluster)  [unwired: 1 in, 3 out]
              n399 = And(x="Cycle Sync Z Correction", y=w844) -> (x .and. y?=w840:bool)
              n400 = Unbundle By Name(w882) -> ("Image Ref"=w877:T4, "Cycle Number"=w862:u16, "Capture?"=w860:bool, "Camera Running?"=w853:bool)
              n401 = call "WFDC Get Current Drift.vi"("Ref Images"=w914, "Z Calibration (slope, inter)"=w913, "Half Shift"=7, "Current Image"=w870, "Error In"=w868, "Track XY Drift?"="Track XY Drift") -> ("Axis 1 Drift (px)"=w835:dbl, "Axis 2 Drift (px)"=w834:dbl, "Z Position (µm)"=w869:dbl, "Error Out"=w867:errorcluster)  [unwired: 6 in]
              "Axis 1 Drift (Pixels)" <- w835
              "Axis 2 Drift (Pixels)" <- w834
              n402 = in-place {
                in-place-border: w869 -> [w955]
                in-place-border: w834 -> [w957]
                in-place-border: w835 -> [w956]
                n403 = in-place-array #2(w908, 0, 1, 2) -> ()  [unwired: 3 out]
                n404 = in-place-array #2(w956, w957, w955) -> (w892:dbl[])  [unwired: 3 out]
              }
              n405 = Select(t=w844, s="Cycle Sync Z Correction", f=TRUE) -> (s? t:f=w845:bool)
              n406 = Index Array(array=w898, index=2) -> (element=w906:dbl)
              n407 = Unbundle By Name(w867) -> ("status"=w864:bool)
              n408 = call "IMAQ Read Custom Data"("error in (no error)"=w858, "Key"="Image Data", "Image"=w877) -> ("error out"=w876:errorcluster, "Custom Data Out"=w879:string)  [unwired: 6 in, 1 out]
              n409 = Unflatten From JSON(JSON string=w879, type and defaults=T26 {"Frame"=0, "Sensor Height"=0, "Sensor Width"=0, "ROI Height"=0, "ROI Width"=0, "ROI Enable?"=FALSE, "Bit per Pixel"=0} ("Camera IMAQ Key Info"), error in (no error)=w876) -> (value=w881:T26, error out=w874:errorcluster)  [unwired: 4 in]
              n410 = Compound Arithmetic op=ADD("Z Position Offset (µm)", w906, w884) -> (w905:dbl)
              n411 = case shown="No Error" w874 {
                tunnel: w881 -> [w921 _]
                tunnel: [w920 u32 0 ("Frame")] -> w875
                tunnel: [w919 u16 0 ("Cycle Number")] -> w861
                tunnel: w862 -> [w919 _]
                tunnel: [w918 w922] -> w859
                tunnel: w860 -> [w918 _]
                tunnel: [w917 w922] -> w852
                tunnel: w853 -> [w917 _]
                frame No Error {
                  n412 = Unbundle By Name(w921) -> ("Frame"=w920:u32)
                }
                frame Error {
                  w922 = FALSE ("Capture?")
                }
              }
              n413 = Subtract(x=w905, y=w869) -> (x-y=w833:dbl)
              "Z Drift Amount" <- w833
              "Z Drift (µm)" <- w833
              n414 = Absolute Value(x=w833) -> (abs(x)=w865:dbl)
              n415 = Greater?(x=w865, y="Z Drift Threshold (µm)") -> (0:w848:bool)
              n416 = Compound Arithmetic op=AND(w848, "Correct Z Drift", w845) -> (w846:bool)
              n417 = Unbundle By Name(w891) -> ("Log Drift?"=w894:bool, "Drift Positions File Ref"=w893:refnum<file>, "Save WF Images?"=w895:bool, "Drift Image File Ref"=w896:refnum<file>)
              n418 = Greater?(x=w865, y="Z Step Correction Limit (µm)") -> (0:w863:bool)
              n419 = case shown="True" w846 {
                tunnel: w897 -> [w947 w954]
                tunnel: w833 -> [_ w951]
                tunnel: [w946 w950] -> w902
                frame False {
                  n420 = call "Stages Messenger.vi"("Stage Notifier Name"=w947, "Actions"=Stage_Actions."Get Position") -> ("Positions"=w946:dbl[])  [unwired: 10 in, 3 out]
                }
                frame True {
                  n421 = Build Array(w951) -> (w953:dbl[])
                  n422 = call "Stages Messenger.vi"("Stage Notifier Name"=w954, "Actions"=Stage_Actions."MVR", "Setpoint"=w953, "Axis"=bool[] [TRUE]) -> ("Positions"=w950:dbl[])  [unwired: 8 in, 3 out]
                }
              }
              n423 = Or(x=w864, y=w863) -> (x .or. y?=w832:bool)
              n424 = case shown="True" w894 {
                tunnel: w895 -> [_ w938]
                tunnel: w893 -> [_ w936]
                tunnel: w896 -> [_ w937]
                tunnel: w870 -> [_ w935]
                tunnel: w869 -> [_ w928]
                tunnel: w833 -> [_ w929]
                tunnel: w835 -> [_ w931]
                tunnel: w834 -> [_ w930]
                tunnel: w875 -> [_ w933]
                tunnel: w861 -> [_ w932]
                tunnel: w859 -> [_ w927]
                tunnel: w852 -> [_ w926]
                frame False {
                }
                frame True {
                  n425 = case shown="True" w938 {
                    tunnel: w937 -> [_ w943]
                    tunnel: w935 -> [_ w942]
                    frame False {
                    }
                    frame True {
                      n426 = Write to Binary File(file (use dialog)=w943, data=w942, 5:FALSE ("prepend array or string size? (T)"), 9:T27."little-endian" ("byte order (0:big-endian, network order)")) -> ()  [unwired: 2 in, 3 out]
                    }
                  }
                  n427 = Format Into String(format string="%d %d %.3f %.3f %.3f %.3f %b %b", w933, w932, w931, w930, w929, w928, w927, w926) -> (resulting string=w925:string)  [unwired: 2 in, 1 out]
                  n428 = Set File Position(offset (in bytes) (0)=i64 0, refnum=w936, from (0:start)=enum16{"start", "end", "current"}."end") -> (refnum out=w939:refnum<file>)  [unwired: 1 in, 1 out]
                  n429 = Write to Text File(file (use dialog)=w939, text=w925) -> ()  [unwired: 2 in, 3 out]
                }
              }
              n430 = Index Array(array=w902, index=0) -> (element=→"Z Stage Position":dbl)
              n431 = And(x="Correct XY Drift", y="Track XY Drift") -> (x .and. y?=w842:bool)
              n432 = Not(x=w842) -> (.not. x?=w841:bool)
              n433 = Select(t=WFDC_Actions."Correct XY Drift" ("x"), s=w842, f=WFDC_Actions."Get Drift / Correct Z") -> (s? t:f=w839:T10)
              n434 = And(x=w841, y=w840) -> (x .and. y?=w837:bool)
              n435 = Select(t=WFDC_Actions."Start Cycle" ("f"), s=w837, f=w839) -> (s? t:f=w836:T10)
              n436 = Select(t=w887, s=w857, f=w836) -> (s? t:f=w856:T10)
              n437 = Select(t=WFDC_Actions."Set Error" ("x"), s=w832, f=w856) -> (s? t:f=w855:T10)
            }
            frame "Correct XY Drift" {
              n438 = Get Notifier Status(notifier=w963) -> (current notification=w970:T9)  [unwired: 1 in, 4 out]
              n439 = Unbundle By Name(w970) -> ("Cycle Sync"=w969:T7)
              n440 = Equal?(x=w969, y=WFDC_Cycle_Pause."Paused") -> (x = y?=w966:bool)
              n441 = Select(t=w966, s="Cycle Sync XY Correction", f=TRUE) -> (s? t:f=w958:bool)
              n442 = case shown="True" w958 {
                tunnel: w964 -> [_ w999]
                tunnel: w971 -> [_ w980]
                tunnel: "Cycle Sync XY Correction" -> [_ w978]
                tunnel: [FALSE w976] -> w960
                frame False {
                }
                frame True {
                  w990 = 7.0 ("y")
                  n443 = Array Subset(array=w999, index=0, length=2) -> (w993:dbl[])
                  n444 = Add(x="XY Drift Threshold (pixels)", y=w990) -> (x+y=w986:dbl)
                  n445 = Subtract(x=w990, y="XY Drift Threshold (pixels)") -> (x-y=w989:dbl)
                  n446 = for {
                    tunnel: w993 -> [w1020] mode=indexing
                    tunnel: [w1019] -> w981 mode=indexing
                    tunnel: w986 -> [w1018]
                    tunnel: w989 -> [w1017]
                    n447 = In Range and Coerce(upper limit=w1018, x=w1020, lower limit=w1017) -> (In Range?=w1019:bool)  [unwired: 1 out]
                  }
                  n448 = And Array Elements(Boolean array=w981) -> (logical AND=w975:bool)
                  n449 = case shown="True" "Flip XY Axis" {
                    tunnel: w993 -> [w1001 w1004]
                    tunnel: w981 -> [w1000 w1005]
                    tunnel: [w1001 w1003] -> w987
                    tunnel: [w1000 w1002] -> w988
                    frame False {
                    }
                    frame True {
                      n450 = Reverse 1D Array(array=w1004) -> (reversed array=w1003:dbl[])
                      n451 = Reverse 1D Array(array=w1005) -> (reversed array=w1002:bool[])
                    }
                  }
                  n452 = And(x=w975, y=w978) -> (x .and. y?=w976:bool)
                  n453 = Build Array("Invert X Axis", "Invert Y Axis") -> (w977:bool[])
                  n454 = for {
                    N: 2 -> [_]
                    tunnel: w988 -> [w1014] mode=indexing
                    tunnel: w987 -> [w1016] mode=indexing
                    tunnel: [w1009] -> w994 mode=indexing
                    tunnel: [w1013] -> w995 mode=indexing
                    tunnel: w986 -> [w1012]
                    tunnel: "XY Drift Step (µm)" -> [w1010]
                    tunnel: w977 -> [w1006] mode=indexing
                    n455 = Greater?(x=w1016, y=w1012) -> (0:w1015:bool)
                    n456 = Negate(x=w1010) -> (-x=w1011:dbl)
                    n457 = Not(x=w1014) -> (.not. x?=w1013:bool)
                    n458 = Select(t=w1010, s=w1015, f=w1011) -> (s? t:f=w1007:dbl)
                    n459 = Negate(x=w1007) -> (-x=w1008:dbl)
                    n460 = Select(t=w1008, s=w1006, f=w1007) -> (s? t:f=w1009:dbl)
                  }
                  n461 = Not(x=w975) -> (.not. x?=→"XY Drift Correction Active":bool)
                  n462 = call "Stages Messenger.vi"("Stage Notifier Name"=w980, "Actions"=Stage_Actions."MVR", "Setpoint"=w994, "Axis"=w995, "Exit While Busy?"=FALSE) -> ()  [unwired: 7 in, 4 out]
                }
              }
              n463 = Select(t=WFDC_Actions."Start Cycle" ("x"), s=w960, f=WFDC_Actions."Get Drift / Correct Z" ("x")) -> (s? t:f=w961:T10)
            }
            frame "Start Cycle" {
              n464 = Get Notifier Status(notifier=w1023) -> (current notification=w1022:T5)  [unwired: 1 in, 4 out]
              n465 = Unbundle By Name(w1022) -> ("Capture?"=w1021:bool)
              n466 = case shown="True" w1021 {
                tunnel: w1024 -> [_ w1034]
                frame False {
                }
                frame True {
                  n467 = Get Notifier Status(notifier=w1034) -> (notifier out=w1035:refnum<notifier>, current notification=w1036:T9)  [unwired: 1 in, 3 out]
                  n468 = Bundle By Name(cluster=w1036, "Cycle Sync"=WFDC_Cycle_Pause."Resume Requested") -> (w1037:T9)
                  n469 = Send Notification(notification=w1037, notifier=w1035) -> (notifier out=w1033:refnum<notifier>)  [unwired: 1 in, 1 out]
                  n470 = while {
                    tunnel: w1033 -> [w1049]
                    tunnel: [w1043] -> w1028
                    i -> [w1047]
                    stop <- w1039 stop-if-true
                    n471 = Wait (ms)(milliseconds to wait=u32 1) -> ()  [unwired: 1 out]
                    n472 = Get Notifier Status(notifier=w1049) -> (notifier out=w1043:refnum<notifier>, current notification=w1044:T9)  [unwired: 1 in, 3 out]
                    n473 = Unbundle By Name(w1044) -> ("Cycle Sync"=w1042:T7)
                    n474 = Greater?(x=w1047, y=4000) -> (0:w1045:bool)
                    n475 = Equal?(x=w1042, y=WFDC_Cycle_Pause."Resumed") -> (x = y?=w1040:bool)
                    n476 = Or(x=w1040, y=w1045) -> (x .or. y?=w1039:bool)
                  }
                  n477 = Get Notifier Status(notifier=w1028) -> (notifier out=w1032:refnum<notifier>, current notification=w1031:T9)  [unwired: 1 in, 3 out]
                  n478 = Bundle By Name(cluster=w1031, "Cycle Sync"=WFDC_Cycle_Pause."Pause Requested") -> (w1030:T9)
                  n479 = Send Notification(notification=w1030, notifier=w1032) -> ()  [unwired: 1 in, 2 out]
                }
              }
            }
            frame "Stop DC", "Set Error" {
              n480 = Equal?(x=w1062, y=WFDC_Actions."Set Error") -> (x = y?=w1054:bool)
              "Error" <- w1054
              n481 = And(x=w1054, y="Abort Capture If Error") -> (x .and. y?=w1059:bool)
              n482 = case shown="True" w1054 {
                frame False {
                }
                frame True {
                  n483 = local write "Setup New"(FALSE ("Setup New")) -> ()
                }
              }
              n484 = Get Notifier Status(notifier=w1074) -> (current notification=w1068:T11)  [unwired: 1 in, 4 out]
              n485 = Select(t=WFDC_Status."Error" ("WFDC Status"), s=w1059, f=WFDC_Status."Idle" ("WFDC Status")) -> (s? t:f=w1057:T8)
              n486 = call "IDS Camera Messenger.vi"("Notifier Name"=w1077, "IDS Actions"=IDS_Actions."Abort") -> ()  [unwired: 8 in, 6 out]
              n487 = Unbundle By Name(w1068) -> ("Ref Images"=w1073:T4[], "Log Drift?"=w1072:bool, "Save WF Images?"=w1070:bool, "Drift Image File Ref"=w1071:refnum<file>, "Drift Positions File Ref"=w1055:refnum<file>)
              n488 = Get Notifier Status(notifier=w1064) -> (notifier out=w1065:refnum<notifier>, current notification=w1066:T9)  [unwired: 1 in, 3 out]
              n489 = Bundle By Name(cluster=w1066, "Cycle Sync"=WFDC_Cycle_Pause."Resumed", "WFDC Status"=w1057) -> (w1067:T9)
              n490 = Send Notification(notification=w1067, notifier=w1065) -> ()  [unwired: 1 in, 2 out]
              n491 = for {
                tunnel: w1073 -> [w1084] mode=indexing
                n492 = call "IMAQ Dispose"("Image"=w1084) -> ()  [unwired: 5 in, 1 out]
              }
              n493 = case shown="True" w1072 {
                tunnel: w1071 -> [_ w1082]
                tunnel: w1055 -> [_ w1081]
                tunnel: w1070 -> [_ w1080]
                frame False {
                }
                frame True {
                  n494 = case shown="True" w1080 {
                    tunnel: w1082 -> [_ w1083]
                    frame False {
                    }
                    frame True {
                      n495 = Close File(refnum=w1083) -> ()  [unwired: 1 in, 2 out]
                    }
                  }
                  n496 = Close File(refnum=w1081) -> ()  [unwired: 1 in, 2 out]
                }
              }
              n497 = property on="Main Tab" class="TabCtl (strict)"() -> ("Pages"=w1053:refnum<vi>[])  [unwired: 2 in, 2 out]
              n498 = Index Array(array=w1053, index=3) -> (element=w1051:refnum<vi>)
              n499 = property class="Page"(reference=w1051, "PageEnb"=T25."Page Enabled" ("Page Enabled State")) -> ()  [unwired: 1 in, 2 out]
            }
            frame "Exit Loop" {
              n500 = local write "Running"(FALSE ("Running")) -> ()
            }
            frame "Quit" {
              n501 = Release Notifier(notifier=w1094, force destroy? (F)=TRUE) -> ()  [unwired: 1 in, 3 out]
              n502 = Release Notifier(notifier=w1093, force destroy? (F)=TRUE) -> ()  [unwired: 1 in, 3 out]
              n503 = Release Notifier(notifier=w1089) -> ()  [unwired: 2 in, 3 out]
            }
          }
        }
      }
      n504 = local write "Quit"(w113) -> ()
    }
  }
